vi "Measurement UI.vi"() -> ()   [LabVIEW 2025, in "Automotive Ethernet Bus Monitor UI.lvlib"]
uses:
  Automotive Ethernet Bus Monitor UI.lvlib
  Protocol Layer.ctl
  <vilib>/gRPC/LabVIEW gRPC Library/Shared/grpcId.ctl
  AETH UI Refs.ctl
  <vilib>/Utility/miscctls.llb/LVRowAndColumnUnsignedTypeDef.ctl
  Table Buffer/Get Status.vi
  Table Buffer/Flush Table.vi
  Table Buffer/Create Buffer.vi
  Table Buffer/Destroy Table Buffer.vi
  OOB gRPC Client/OOB gRPC Client.lvlib
  <vilib>/gRPC/LabVIEW gRPC Library/grpc-lvsupport-release.lvlib
panel:
  in  "HELP":bool
  out "IsRestarting?":bool
  out "New Data?":bool
  in  "Clear Packets":bool
  in  "SAVE FORMAT":u16(ring) items=["TDMS", "CSV"]
  in  "INTERFACE NAME":refnum<k21>
  out "TC10 POWER MODE":bool
  in  "TC10":bool
  out "Latest Error":string
  out "STATUS":string
  in  "PAUSE":bool
  out "CAPTURING STREAM":bool
  in  "INTERFACE NAME STRING":string
  in  "ETHERNET MODE IN":i32(ring) items=["Automotive Ethernet", "Standard Ethernet"]
  in  "SAVE TO CSV":bool
  in  "SORT BY":u16(ring) items=["Packet_Number", "Timestamp", "Source", "Destination", "Protocol", "Length", "Data"]
  in  "PATH":path
  in  "FILTER STRING":string
  out "FULL PACKET":string
  out "Packets":string[][](table)=[["10", "11/14/2025 1:57:47 PM", "10.0.0.1", "10.0.0.2", "UDP", "0.821211", "thisisdata"], ["100", "11/14/2025 1:57:47 PM", "10.0.0.1", "10.0.0.2", "UDP", "0.956516", "thisisdata"], ["1002", "11/14/2025 1:57:47 PM", "10.0.0.1", "10.0.0.2", "UDP", "0.960987", "thisisdata"], ["1007", "11/14/2025 1:57:47 PM", "10.0.0.1", "10.0.0.2", "UDP", "0.867598", "thisisdata"], ["1009", "11/14/2025 1:57:47 PM", "10.0.0.1", "10.0.0.2", "UDP", "0.839638", "thisisdata"], ["101", "11/14/2025 1:57:47 PM", "10.0.0.1", "10.0.0.2", "UDP", "0.891709", "thisisdata"], ["1012", "11/14/2025 1:57:47 PM", "10.0.0.1", "10.0.0.2", "UDP", "0.969576", "thisisdata"], ["1017", "11/14/2025 1:57:47 PM", "10.0.0.1", "10.0.0.2", "UDP", "0.871748", "thisisdata"], ["1021", "11/14/2025 1:57:47 PM", "10.0.0.1", "10.0.0.2", "UDP", "0.904588", "thisisdata"], ["1026", "11/14/2025 1:57:47 PM", "10.0.0.1", "10.0.0.2", "UDP", "0.986150", "thisisdata"], ["1027", "11/14/2025 1:57:47 PM", "10.0.0.1", "10.0.0.2", "UDP", "0.775009", "thisisdata"], ["1028", "11/14/2025 1:57:47 PM", "10.0.0.1", "10.0.0.2", "UDP", "0.817026", "thisisdata"], ["1036", "11/14/2025 1:57:47 PM", "10.0.0.1", "10.0.0.2", "UDP", "0.839495", "thisisdata"], ["1038", "11/14/2025 1:57:47 PM", "10.0.0.1", "10.0.0.2", "UDP", "0.847314", "thisisdata"], ["1044", "11/14/2025 1:57:47 PM", "10.0.0.1", "10.0.0.2", "UDP", "0.793260", "thisisdata"], ["1048", "11/14/2025 1:57:47 PM", "10.0.0.1", "10.0.0.2", "UDP", "0.742047", "thisisdata"], ["1049", "11/14/2025 1:57:47 PM", "10.0.0.1", "10.0.0.2", "UDP", "0.771430", "thisisdata"], ["1051", "11/14/2025 1:57:47 PM", "10.0.0.1", "10.0.0.2", "UDP", "0.889463", "thisisdata"], ["1052", "11/14/2025 1:57:47 PM", "10.0.0.1", "10.0.0.2", "UDP", "0.702476", "thisisdata"], ["1053", "11/14/2025 1:57:47 PM", "10.0.0.1", "10.0.0.2", "UDP", "0.943543", "thisisdata"], ["1055", "11/14/2025 1:57:47 PM", "10.0.0.1", "10.0.0.2", "UDP", "0.912358", "thisisdata"], ["1062", "11/14/2025 1:57:47 PM", "10.0.0.1", "10.0.0.2", "UDP", "0.883876", "thisisdata"], ["1065", "11/14/2025 1:57:47 PM", "10.0.0.1", "10.0.0.2", "UDP", "0.998758", "thisisdata"], ["1066", "11/14/2025 1:57:47 PM", "10.0.0.1", "10.0.0.2", "UDP", "0.980816", "thisisdata"], ["1067", "11/14/2025 1:57:47 PM", "10.0.0.1", "10.0.0.2", "UDP", "0.862874", "thisisdata"], ["1074", "11/14/2025 1:57:47 PM", "10.0.0.1", "10.0.0.2", "UDP", "0.985200", "thisisdata"], ["1075", "11/14/2025 1:57:47 PM", "10.0.0.1", "10.0.0.2", "UDP", "0.895925", "thisisdata"], ["108", "11/14/2025 1:57:47 PM", "10.0.0.1", "10.0.0.2", "UDP", "0.746068", "thisisdata"], ["1083", "11/14/2025 1:57:47 PM", "10.0.0.1", "10.0.0.2", "UDP", "0.976636", "thisisdata"], ["1084", "11/14/2025 1:57:47 PM", "10.0.0.1", "10.0.0.2", "UDP", "0.746952", "thisisdata"], ["1086", "11/14/2025 1:57:47 PM", "10.0.0.1", "10.0.0.2", "UDP", "0.772755", "thisisdata"], ["1088", "11/14/2025 1:57:47 PM", "10.0.0.1", "10.0.0.2", "UDP", "0.942784", "thisisdata"], ["1090", "11/14/2025 1:57:47 PM", "10.0.0.1", "10.0.0.2", "UDP", "0.927067", "thisisdata"], ["1092", "11/14/2025 1:57:47 PM", "10.0.0.1", "10.0.0.2", "UDP", "0.875037", "thisisdata"], ["11", "11/14/2025 1:57:47 PM", "10.0.0.1", "10.0.0.2", "UDP", "0.939175", "thisisdata"], ["1101", "11/14/2025 1:57:47 PM", "10.0.0.1", "10.0.0.2", "UDP", "0.730371", "thisisdata"], ["1102", "11/14/2025 1:57:47 PM", "10.0.0.1", "10.0.0.2", "UDP", "0.711041", "thisisdata"], ["1103", "11/14/2025 1:57:47 PM", "10.0.0.1", "10.0.0.2", "UDP", "0.802089", "thisisdata"], ["1104", "11/14/2025 1:57:47 PM", "10.0.0.1", "10.0.0.2", "UDP", "0.975316", "thisisdata"], ["1108", "11/14/2025 1:57:47 PM", "10.0.0.1", "10.0.0.2", "UDP", "0.840307", "thisisdata"], ["1111", "11/14/2025 1:57:47 PM", "10.0.0.1", "10.0.0.2", "UDP", "0.734069", "thisisdata"], ["1113", "11/14/2025 1:57:47 PM", "10.0.0.1", "10.0.0.2", "UDP", "0.897764", "thisisdata"], ["1114", "11/14/2025 1:57:47 PM", "10.0.0.1", "10.0.0.2", "UDP", "0.704577", "thisisdata"], ["1115", "11/14/2025 1:57:47 PM", "10.0.0.1", "10.0.0.2", "UDP", "0.831595", "thisisdata"], ["1123", "11/14/2025 1:57:47 PM", "10.0.0.1", "10.0.0.2", "UDP", "0.869848", "thisisdata"], ["1130", "11/14/2025 1:57:47 PM", "10.0.0.1", "10.0.0.2", "UDP", "0.848458", "thisisdata"], ["1131", "11/14/2025 1:57:47 PM", "10.0.0.1", "10.0.0.2", "UDP", "0.914476", "thisisdata"], ["1139", "11/14/2025 1:57:47 PM", "10.0.0.1", "10.0.0.2", "UDP", "0.851881", "thisisdata"], ["1142", "11/14/2025 1:57:47 PM", "10.0.0.1", "10.0.0.2", "UDP", "0.781918", "thisisdata"], ["1148", "11/14/2025 1:57:47 PM", "10.0.0.1", "10.0.0.2", "UDP", "0.839308", "thisisdata"], ["115", "11/14/2025 1:57:47 PM", "10.0.0.1", "10.0.0.2", "UDP", "0.824463", "thisisdata"], ["1153", "11/14/2025 1:57:47 PM", "10.0.0.1", "10.0.0.2", "UDP", "0.762073", "thisisdata"], ["116", "11/14/2025 1:57:47 PM", "10.0.0.1", "10.0.0.2", "UDP", "0.718284", "thisisdata"], ["1164", "11/14/2025 1:57:47 PM", "10.0.0.1", "10.0.0.2", "UDP", "0.901802", "thisisdata"], ["1165", "11/14/2025 1:57:47 PM", "10.0.0.1", "10.0.0.2", "UDP", "0.782467", "thisisdata"], ["1168", "11/14/2025 1:57:47 PM", "10.0.0.1", "10.0.0.2", "UDP", "0.901873", "thisisdata"], ["1177", "11/14/2025 1:57:47 PM", "10.0.0.1", "10.0.0.2", "UDP", "0.889595", "thisisdata"], ["118", "11/14/2025 1:57:47 PM", "10.0.0.1", "10.0.0.2", "UDP", "0.966309", "thisisdata"], ["1181", "11/14/2025 1:57:47 PM", "10.0.0.1", "10.0.0.2", "UDP", "0.741139", "thisisdata"], ["1182", "11/14/2025 1:57:47 PM", "10.0.0.1", "10.0.0.2", "UDP", "0.954023", "thisisdata"], ["1183", "11/14/2025 1:57:47 PM", "10.0.0.1", "10.0.0.2", "UDP", "0.881562", "thisisdata"], ["1184", "11/14/2025 1:57:47 PM", "10.0.0.1", "10.0.0.2", "UDP", "0.852993", "thisisdata"], ["1185", "11/14/2025 1:57:47 PM", "10.0.0.1", "10.0.0.2", "UDP", "0.885773", "thisisdata"], ["1187", "11/14/2025 1:57:47 PM", "10.0.0.1", "10.0.0.2", "UDP", "0.801737", "thisisdata"], ["1195", "11/14/2025 1:57:47 PM", "10.0.0.1", "10.0.0.2", "UDP", "0.790347", "thisisdata"], ["1196", "11/14/2025 1:57:47 PM", "10.0.0.1", "10.0.0.2", "UDP", "0.864754", "thisisdata"], ["1197", "11/14/2025 1:57:47 PM", "10.0.0.1", "10.0.0.2", "UDP", "0.709221", "thisisdata"], ["121", "11/14/2025 1:57:47 PM", "10.0.0.1", "10.0.0.2", "UDP", "0.913497", "thisisdata"], ["1211", "11/14/2025 1:57:47 PM", "10.0.0.1", "10.0.0.2", "UDP", "0.965122", "thisisdata"], ["1213", "11/14/2025 1:57:47 PM", "10.0.0.1", "10.0.0.2", "UDP", "0.973075", "thisisdata"], ["1218", "11/14/2025 1:57:47 PM", "10.0.0.1", "10.0.0.2", "UDP", "0.904226", "thisisdata"], ["1222", "11/14/2025 1:57:47 PM", "10.0.0.1", "10.0.0.2", "UDP", "0.828121", "thisisdata"], ["1225", "11/14/2025 1:57:47 PM", "10.0.0.1", "10.0.0.2", "UDP", "0.730012", "thisisdata"], ["1226", "11/14/2025 1:57:47 PM", "10.0.0.1", "10.0.0.2", "UDP", "0.762505", "thisisdata"], ["123", "11/14/2025 1:57:47 PM", "10.0.0.1", "10.0.0.2", "UDP", "0.900157", "thisisdata"], ["1230", "11/14/2025 1:57:47 PM", "10.0.0.1", "10.0.0.2", "UDP", "0.958830", "thisisdata"], ["1231", "11/14/2025 1:57:47 PM", "10.0.0.1", "10.0.0.2", "UDP", "0.727490", "thisisdata"], ["1232", "11/14/2025 1:57:47 PM", "10.0.0.1", "10.0.0.2", "UDP", "0.913030", "thisisdata"], ["1234", "11/14/2025 1:57:47 PM", "10.0.0.1", "10.0.0.2", "UDP", "0.711353", "thisisdata"], ["1237", "11/14/2025 1:57:47 PM", "10.0.0.1", "10.0.0.2", "UDP", "0.704839", "thisisdata"], ["1240", "11/14/2025 1:57:47 PM", "10.0.0.1", "10.0.0.2", "UDP", "0.808493", "thisisdata"], ["1241", "11/14/2025 1:57:47 PM", "10.0.0.1", "10.0.0.2", "UDP", "0.750334", "thisisdata"], ["1242", "11/14/2025 1:57:47 PM", "10.0.0.1", "10.0.0.2", "UDP", "0.953795", "thisisdata"], ["1243", "11/14/2025 1:57:47 PM", "10.0.0.1", "10.0.0.2", "UDP", "0.914837", "thisisdata"], ["125", "11/14/2025 1:57:47 PM", "10.0.0.1", "10.0.0.2", "UDP", "0.850827", "thisisdata"], ["1252", "11/14/2025 1:57:47 PM", "10.0.0.1", "10.0.0.2", "UDP", "0.889690", "thisisdata"], ["1253", "11/14/2025 1:57:47 PM", "10.0.0.1", "10.0.0.2", "UDP", "0.800545", "thisisdata"], ["1255", "11/14/2025 1:57:47 PM", "10.0.0.1", "10.0.0.2", "UDP", "0.813802", "thisisdata"], ["1262", "11/14/2025 1:57:47 PM", "10.0.0.1", "10.0.0.2", "UDP", "0.882839", "thisisdata"], ["1265", "11/14/2025 1:57:47 PM", "10.0.0.1", "10.0.0.2", "UDP", "0.898409", "thisisdata"], ["127", "11/14/2025 1:57:47 PM", "10.0.0.1", "10.0.0.2", "UDP", "0.713807", "thisisdata"], ["1275", "11/14/2025 1:57:47 PM", "10.0.0.1", "10.0.0.2", "UDP", "0.972156", "thisisdata"], ["1284", "11/14/2025 1:57:47 PM", "10.0.0.1", "10.0.0.2", "UDP", "0.978269", "thisisdata"], ["1289", "11/14/2025 1:57:47 PM", "10.0.0.1", "10.0.0.2", "UDP", "0.740155", "thisisdata"], ["1299", "11/14/2025 1:57:47 PM", "10.0.0.1", "10.0.0.2", "UDP", "0.953843", "thisisdata"], ["13", "11/14/2025 1:57:47 PM", "10.0.0.1", "10.0.0.2", "UDP", "0.842815", "thisisdata"], ["1301", "11/14/2025 1:57:47 PM", "10.0.0.1", "10.0.0.2", "UDP", "0.879611", "thisisdata"], ["1302", "11/14/2025 1:57:47 PM", "10.0.0.1", "10.0.0.2", "UDP", "0.945983", "thisisdata"], ["1303", "11/14/2025 1:57:47 PM", "10.0.0.1", "10.0.0.2", "UDP", "0.755170", "thisisdata"], ["1307", "11/14/2025 1:57:47 PM", "10.0.0.1", "10.0.0.2", "UDP", "0.773780", "thisisdata"], ["1312", "11/14/2025 1:57:47 PM", "10.0.0.1", "10.0.0.2", "UDP", "0.814087", "thisisdata"], ["1314", "11/14/2025 1:57:47 PM", "10.0.0.1", "10.0.0.2", "UDP", "0.980063", "thisisdata"], ["1317", "11/14/2025 1:57:47 PM", "10.0.0.1", "10.0.0.2", "UDP", "0.829011", "thisisdata"], ["1320", "11/14/2025 1:57:47 PM", "10.0.0.1", "10.0.0.2", "UDP", "0.758120", "thisisdata"], ["1321", "11/14/2025 1:57:47 PM", "10.0.0.1", "10.0.0.2", "UDP", "0.759463", "thisisdata"], ["1322", "11/14/2025 1:57:47 PM", "10.0.0.1", "10.0.0.2", "UDP", "0.824116", "thisisdata"], ["1323", "11/14/2025 1:57:47 PM", "10.0.0.1", "10.0.0.2", "UDP", "0.762172", "thisisdata"], ["1324", "11/14/2025 1:57:47 PM", "10.0.0.1", "10.0.0.2", "UDP", "0.885589", "thisisdata"], ["1330", "11/14/2025 1:57:47 PM", "10.0.0.1", "10.0.0.2", "UDP", "0.942420", "thisisdata"], ["1333", "11/14/2025 1:57:47 PM", "10.0.0.1", "10.0.0.2", "UDP", "0.798878", "thisisdata"], ["1338", "11/14/2025 1:57:47 PM", "10.0.0.1", "10.0.0.2", "UDP", "0.748441", "thisisdata"], ["134", "11/14/2025 1:57:47 PM", "10.0.0.1", "10.0.0.2", "UDP", "0.739118", "thisisdata"], ["1341", "11/14/2025 1:57:47 PM", "10.0.0.1", "10.0.0.2", "UDP", "0.912641", "thisisdata"], ["1342", "11/14/2025 1:57:47 PM", "10.0.0.1", "10.0.0.2", "UDP", "0.833794", "thisisdata"], ["1346", "11/14/2025 1:57:47 PM", "10.0.0.1", "10.0.0.2", "UDP", "0.938173", "thisisdata"], ["1348", "11/14/2025 1:57:47 PM", "10.0.0.1", "10.0.0.2", "UDP", "0.703225", "thisisdata"], ["1349", "11/14/2025 1:57:47 PM", "10.0.0.1", "10.0.0.2", "UDP", "0.962230", "thisisdata"], ["1351", "11/14/2025 1:57:47 PM", "10.0.0.1", "10.0.0.2", "UDP", "0.923262", "thisisdata"], ["1357", "11/14/2025 1:57:47 PM", "10.0.0.1", "10.0.0.2", "UDP", "0.977014", "thisisdata"], ["1358", "11/14/2025 1:57:47 PM", "10.0.0.1", "10.0.0.2", "UDP", "0.904471", "thisisdata"], ["1360", "11/14/2025 1:57:47 PM", "10.0.0.1", "10.0.0.2", "UDP", "0.840541", "thisisdata"], ["1364", "11/14/2025 1:57:47 PM", "10.0.0.1", "10.0.0.2", "UDP", "0.759527", "thisisdata"], ["1367", "11/14/2025 1:57:47 PM", "10.0.0.1", "10.0.0.2", "UDP", "0.926483", "thisisdata"], ["1369", "11/14/2025 1:57:47 PM", "10.0.0.1", "10.0.0.2", "UDP", "0.897696", "thisisdata"], ["1371", "11/14/2025 1:57:47 PM", "10.0.0.1", "10.0.0.2", "UDP", "0.987694", "thisisdata"], ["1374", "11/14/2025 1:57:47 PM", "10.0.0.1", "10.0.0.2", "UDP", "0.795706", "thisisdata"], ["1377", "11/14/2025 1:57:47 PM", "10.0.0.1", "10.0.0.2", "UDP", "0.927883", "thisisdata"], ["1378", "11/14/2025 1:57:47 PM", "10.0.0.1", "10.0.0.2", "UDP", "0.986175", "thisisdata"], ["1379", "11/14/2025 1:57:47 PM", "10.0.0.1", "10.0.0.2", "UDP", "0.716053", "thisisdata"], ["138", "11/14/2025 1:57:47 PM", "10.0.0.1", "10.0.0.2", "UDP", "0.961495", "thisisdata"], ["1381", "11/14/2025 1:57:47 PM", "10.0.0.1", "10.0.0.2", "UDP", "0.839552", "thisisdata"], ["1382", "11/14/2025 1:57:47 PM", "10.0.0.1", "10.0.0.2", "UDP", "0.914187", "thisisdata"], ["1388", "11/14/2025 1:57:47 PM", "10.0.0.1", "10.0.0.2", "UDP", "0.890783", "thisisdata"], ["1390", "11/14/2025 1:57:47 PM", "10.0.0.1", "10.0.0.2", "UDP", "0.913426", "thisisdata"], ["1391", "11/14/2025 1:57:47 PM", "10.0.0.1", "10.0.0.2", "UDP", "0.758421", "thisisdata"], ["1394", "11/14/2025 1:57:47 PM", "10.0.0.1", "10.0.0.2", "UDP", "0.884168", "thisisdata"], ["1395", "11/14/2025 1:57:47 PM", "10.0.0.1", "10.0.0.2", "UDP", "0.773979", "thisisdata"], ["1397", "11/14/2025 1:57:47 PM", "10.0.0.1", "10.0.0.2", "UDP", "0.827235", "thisisdata"], ["14", "11/14/2025 1:57:47 PM", "10.0.0.1", "10.0.0.2", "UDP", "0.839466", "thisisdata"], ["1403", "11/14/2025 1:57:47 PM", "10.0.0.1", "10.0.0.2", "UDP", "0.889704", "thisisdata"], ["1411", "11/14/2025 1:57:47 PM", "10.0.0.1", "10.0.0.2", "UDP", "0.967881", "thisisdata"], ["1417", "11/14/2025 1:57:47 PM", "10.0.0.1", "10.0.0.2", "UDP", "0.962037", "thisisdata"], ["1418", "11/14/2025 1:57:47 PM", "10.0.0.1", "10.0.0.2", "UDP", "0.951923", "thisisdata"], ["1419", "11/14/2025 1:57:47 PM", "10.0.0.1", "10.0.0.2", "UDP", "0.912131", "thisisdata"], ["142", "11/14/2025 1:57:47 PM", "10.0.0.1", "10.0.0.2", "UDP", "0.900485", "thisisdata"], ["1421", "11/14/2025 1:57:47 PM", "10.0.0.1", "10.0.0.2", "UDP", "0.972293", "thisisdata"], ["1428", "11/14/2025 1:57:47 PM", "10.0.0.1", "10.0.0.2", "UDP", "0.706623", "thisisdata"], ["143", "11/14/2025 1:57:47 PM", "10.0.0.1", "10.0.0.2", "UDP", "0.862774", "thisisdata"], ["1430", "11/14/2025 1:57:47 PM", "10.0.0.1", "10.0.0.2", "UDP", "0.831932", "thisisdata"], ["1432", "11/14/2025 1:57:47 PM", "10.0.0.1", "10.0.0.2", "UDP", "0.955880", "thisisdata"], ["1434", "11/14/2025 1:57:47 PM", "10.0.0.1", "10.0.0.2", "UDP", "0.885487", "thisisdata"], ["1436", "11/14/2025 1:57:47 PM", "10.0.0.1", "10.0.0.2", "UDP", "0.804128", "thisisdata"], ["144", "11/14/2025 1:57:47 PM", "10.0.0.1", "10.0.0.2", "UDP", "0.837449", "thisisdata"], ["1440", "11/14/2025 1:57:47 PM", "10.0.0.1", "10.0.0.2", "UDP", "0.973148", "thisisdata"], ["1447", "11/14/2025 1:57:47 PM", "10.0.0.1", "10.0.0.2", "UDP", "0.718230", "thisisdata"], ["1449", "11/14/2025 1:57:47 PM", "10.0.0.1", "10.0.0.2", "UDP", "0.724932", "thisisdata"], ["145", "11/14/2025 1:57:47 PM", "10.0.0.1", "10.0.0.2", "UDP", "0.834936", "thisisdata"], ["1453", "11/14/2025 1:57:47 PM", "10.0.0.1", "10.0.0.2", "UDP", "0.709100", "thisisdata"], ["1457", "11/14/2025 1:57:47 PM", "10.0.0.1", "10.0.0.2", "UDP", "0.785225", "thisisdata"], ["146", "11/14/2025 1:57:47 PM", "10.0.0.1", "10.0.0.2", "UDP", "0.967161", "thisisdata"], ["1467", "11/14/2025 1:57:47 PM", "10.0.0.1", "10.0.0.2", "UDP", "0.721965", "thisisdata"], ["1468", "11/14/2025 1:57:47 PM", "10.0.0.1", "10.0.0.2", "UDP", "0.994270", "thisisdata"], ["1469", "11/14/2025 1:57:47 PM", "10.0.0.1", "10.0.0.2", "UDP", "0.848087", "thisisdata"], ["147", "11/14/2025 1:57:47 PM", "10.0.0.1", "10.0.0.2", "UDP", "0.777765", "thisisdata"], ["1473", "11/14/2025 1:57:47 PM", "10.0.0.1", "10.0.0.2", "UDP", "0.959502", "thisisdata"], ["1474", "11/14/2025 1:57:47 PM", "10.0.0.1", "10.0.0.2", "UDP", "0.934426", "thisisdata"], ["1475", "11/14/2025 1:57:47 PM", "10.0.0.1", "10.0.0.2", "UDP", "0.755909", "thisisdata"], ["1480", "11/14/2025 1:57:47 PM", "10.0.0.1", "10.0.0.2", "UDP", "0.947402", "thisisdata"], ["1482", "11/14/2025 1:57:47 PM", "10.0.0.1", "10.0.0.2", "UDP", "0.966904", "thisisdata"], ["1488", "11/14/2025 1:57:47 PM", "10.0.0.1", "10.0.0.2", "UDP", "0.717426", "thisisdata"], ["1494", "11/14/2025 1:57:47 PM", "10.0.0.1", "10.0.0.2", "UDP", "0.937831", "thisisdata"], ["1496", "11/14/2025 1:57:47 PM", "10.0.0.1", "10.0.0.2", "UDP", "0.872401", "thisisdata"], ["1497", "11/14/2025 1:57:47 PM", "10.0.0.1", "10.0.0.2", "UDP", "0.814240", "thisisdata"], ["1498", "11/14/2025 1:57:47 PM", "10.0.0.1", "10.0.0.2", "UDP", "0.750281", "thisisdata"], ["151", "11/14/2025 1:57:47 PM", "10.0.0.1", "10.0.0.2", "UDP", "0.875864", "thisisdata"], ["152", "11/14/2025 1:57:47 PM", "10.0.0.1", "10.0.0.2", "UDP", "0.771317", "thisisdata"], ["153", "11/14/2025 1:57:47 PM", "10.0.0.1", "10.0.0.2", "UDP", "0.839422", "thisisdata"], ["156", "11/14/2025 1:57:47 PM", "10.0.0.1", "10.0.0.2", "UDP", "0.729712", "thisisdata"], ["158", "11/14/2025 1:57:47 PM", "10.0.0.1", "10.0.0.2", "UDP", "0.878224", "thisisdata"], ["159", "11/14/2025 1:57:47 PM", "10.0.0.1", "10.0.0.2", "UDP", "0.963331", "thisisdata"], ["16", "11/14/2025 1:57:47 PM", "10.0.0.1", "10.0.0.2", "UDP", "0.706402", "thisisdata"], ["160", "11/14/2025 1:57:47 PM", "10.0.0.1", "10.0.0.2", "UDP", "0.803364", "thisisdata"], ["161", "11/14/2025 1:57:47 PM", "10.0.0.1", "10.0.0.2", "UDP", "0.841035", "thisisdata"], ["162", "11/14/2025 1:57:47 PM", "10.0.0.1", "10.0.0.2", "UDP", "0.815937", "thisisdata"], ["171", "11/14/2025 1:57:47 PM", "10.0.0.1", "10.0.0.2", "UDP", "0.923770", "thisisdata"], ["175", "11/14/2025 1:57:47 PM", "10.0.0.1", "10.0.0.2", "UDP", "0.775138", "thisisdata"], ["182", "11/14/2025 1:57:47 PM", "10.0.0.1", "10.0.0.2", "UDP", "0.769656", "thisisdata"], ["183", "11/14/2025 1:57:47 PM", "10.0.0.1", "10.0.0.2", "UDP", "0.886119", "thisisdata"], ["184", "11/14/2025 1:57:47 PM", "10.0.0.1", "10.0.0.2", "UDP", "0.717707", "thisisdata"], ["186", "11/14/2025 1:57:47 PM", "10.0.0.1", "10.0.0.2", "UDP", "0.963742", "thisisdata"], ["189", "11/14/2025 1:57:47 PM", "10.0.0.1", "10.0.0.2", "UDP", "0.822883", "thisisdata"], ["204", "11/14/2025 1:57:47 PM", "10.0.0.1", "10.0.0.2", "UDP", "0.812997", "thisisdata"], ["211", "11/14/2025 1:57:47 PM", "10.0.0.1", "10.0.0.2", "UDP", "0.819247", "thisisdata"], ["215", "11/14/2025 1:57:47 PM", "10.0.0.1", "10.0.0.2", "UDP", "0.723501", "thisisdata"], ["218", "11/14/2025 1:57:47 PM", "10.0.0.1", "10.0.0.2", "UDP", "0.817730", "thisisdata"], ["222", "11/14/2025 1:57:47 PM", "10.0.0.1", "10.0.0.2", "UDP", "0.952346", "thisisdata"], ["225", "11/14/2025 1:57:47 PM", "10.0.0.1", "10.0.0.2", "UDP", "0.939892", "thisisdata"], ["226", "11/14/2025 1:57:47 PM", "10.0.0.1", "10.0.0.2", "UDP", "0.992709", "thisisdata"], ["235", "11/14/2025 1:57:47 PM", "10.0.0.1", "10.0.0.2", "UDP", "0.941276", "thisisdata"], ["246", "11/14/2025 1:57:47 PM", "10.0.0.1", "10.0.0.2", "UDP", "0.904690", "thisisdata"], ["25", "11/14/2025 1:57:47 PM", "10.0.0.1", "10.0.0.2", "UDP", "0.910103", "thisisdata"], ["251", "11/14/2025 1:57:47 PM", "10.0.0.1", "10.0.0.2", "UDP", "0.720603", "thisisdata"], ["252", "11/14/2025 1:57:47 PM", "10.0.0.1", "10.0.0.2", "UDP", "0.978412", "thisisdata"], ["253", "11/14/2025 1:57:47 PM", "10.0.0.1", "10.0.0.2", "UDP", "0.859802", "thisisdata"], ["257", "11/14/2025 1:57:47 PM", "10.0.0.1", "10.0.0.2", "UDP", "0.706716", "thisisdata"], ["265", "11/14/2025 1:57:47 PM", "10.0.0.1", "10.0.0.2", "UDP", "0.954216", "thisisdata"], ["266", "11/14/2025 1:57:47 PM", "10.0.0.1", "10.0.0.2", "UDP", "0.978586", "thisisdata"], ["268", "11/14/2025 1:57:47 PM", "10.0.0.1", "10.0.0.2", "UDP", "0.728359", "thisisdata"], ["269", "11/14/2025 1:57:47 PM", "10.0.0.1", "10.0.0.2", "UDP", "0.805801", "thisisdata"], ["27", "11/14/2025 1:57:47 PM", "10.0.0.1", "10.0.0.2", "UDP", "0.890670", "thisisdata"], ["270", "11/14/2025 1:57:47 PM", "10.0.0.1", "10.0.0.2", "UDP", "0.730876", "thisisdata"], ["271", "11/14/2025 1:57:47 PM", "10.0.0.1", "10.0.0.2", "UDP", "0.964321", "thisisdata"], ["273", "11/14/2025 1:57:47 PM", "10.0.0.1", "10.0.0.2", "UDP", "0.822445", "thisisdata"], ["280", "11/14/2025 1:57:47 PM", "10.0.0.1", "10.0.0.2", "UDP", "0.805915", "thisisdata"], ["282", "11/14/2025 1:57:47 PM", "10.0.0.1", "10.0.0.2", "UDP", "0.995119", "thisisdata"], ["285", "11/14/2025 1:57:47 PM", "10.0.0.1", "10.0.0.2", "UDP", "0.702493", "thisisdata"], ["287", "11/14/2025 1:57:47 PM", "10.0.0.1", "10.0.0.2", "UDP", "0.895930", "thisisdata"], ["293", "11/14/2025 1:57:47 PM", "10.0.0.1", "10.0.0.2", "UDP", "0.782899", "thisisdata"], ["30", "11/14/2025 1:57:47 PM", "10.0.0.1", "10.0.0.2", "UDP", "0.919602", "thisisdata"], ["302", "11/14/2025 1:57:47 PM", "10.0.0.1", "10.0.0.2", "UDP", "0.702472", "thisisdata"], ["303", "11/14/2025 1:57:47 PM", "10.0.0.1", "10.0.0.2", "UDP", "0.776732", "thisisdata"], ["304", "11/14/2025 1:57:47 PM", "10.0.0.1", "10.0.0.2", "UDP", "0.805126", "thisisdata"], ["305", "11/14/2025 1:57:47 PM", "10.0.0.1", "10.0.0.2", "UDP", "0.974208", "thisisdata"], ["306", "11/14/2025 1:57:47 PM", "10.0.0.1", "10.0.0.2", "UDP", "0.799271", "thisisdata"], ["307", "11/14/2025 1:57:47 PM", "10.0.0.1", "10.0.0.2", "UDP", "0.985518", "thisisdata"], ["310", "11/14/2025 1:57:47 PM", "10.0.0.1", "10.0.0.2", "UDP", "0.995978", "thisisdata"], ["311", "11/14/2025 1:57:47 PM", "10.0.0.1", "10.0.0.2", "UDP", "0.987227", "thisisdata"], ["312", "11/14/2025 1:57:47 PM", "10.0.0.1", "10.0.0.2", "UDP", "0.797511", "thisisdata"], ["314", "11/14/2025 1:57:47 PM", "10.0.0.1", "10.0.0.2", "UDP", "0.838158", "thisisdata"], ["316", "11/14/2025 1:57:47 PM", "10.0.0.1", "10.0.0.2", "UDP", "0.898183", "thisisdata"], ["319", "11/14/2025 1:57:47 PM", "10.0.0.1", "10.0.0.2", "UDP", "0.813462", "thisisdata"], ["320", "11/14/2025 1:57:47 PM", "10.0.0.1", "10.0.0.2", "UDP", "0.725049", "thisisdata"], ["322", "11/14/2025 1:57:47 PM", "10.0.0.1", "10.0.0.2", "UDP", "0.954221", "thisisdata"], ["324", "11/14/2025 1:57:47 PM", "10.0.0.1", "10.0.0.2", "UDP", "0.773913", "thisisdata"], ["330", "11/14/2025 1:57:47 PM", "10.0.0.1", "10.0.0.2", "UDP", "0.846395", "thisisdata"], ["331", "11/14/2025 1:57:47 PM", "10.0.0.1", "10.0.0.2", "UDP", "0.868667", "thisisdata"], ["333", "11/14/2025 1:57:47 PM", "10.0.0.1", "10.0.0.2", "UDP", "0.915934", "thisisdata"], ["335", "11/14/2025 1:57:47 PM", "10.0.0.1", "10.0.0.2", "UDP", "0.744820", "thisisdata"], ["344", "11/14/2025 1:57:47 PM", "10.0.0.1", "10.0.0.2", "UDP", "0.737303", "thisisdata"], ["345", "11/14/2025 1:57:47 PM", "10.0.0.1", "10.0.0.2", "UDP", "0.744197", "thisisdata"], ["347", "11/14/2025 1:57:47 PM", "10.0.0.1", "10.0.0.2", "UDP", "0.816133", "thisisdata"], ["35", "11/14/2025 1:57:47 PM", "10.0.0.1", "10.0.0.2", "UDP", "0.980754", "thisisdata"], ["359", "11/14/2025 1:57:47 PM", "10.0.0.1", "10.0.0.2", "UDP", "0.710696", "thisisdata"], ["36", "11/14/2025 1:57:47 PM", "10.0.0.1", "10.0.0.2", "UDP", "0.821418", "thisisdata"], ["361", "11/14/2025 1:57:47 PM", "10.0.0.1", "10.0.0.2", "UDP", "0.810013", "thisisdata"], ["369", "11/14/2025 1:57:47 PM", "10.0.0.1", "10.0.0.2", "UDP", "0.918693", "thisisdata"], ["373", "11/14/2025 1:57:47 PM", "10.0.0.1", "10.0.0.2", "UDP", "0.860255", "thisisdata"], ["376", "11/14/2025 1:57:47 PM", "10.0.0.1", "10.0.0.2", "UDP", "0.749631", "thisisdata"], ["38", "11/14/2025 1:57:47 PM", "10.0.0.1", "10.0.0.2", "UDP", "0.844976", "thisisdata"], ["383", "11/14/2025 1:57:47 PM", "10.0.0.1", "10.0.0.2", "UDP", "0.800813", "thisisdata"], ["384", "11/14/2025 1:57:47 PM", "10.0.0.1", "10.0.0.2", "UDP", "0.765681", "thisisdata"], ["391", "11/14/2025 1:57:47 PM", "10.0.0.1", "10.0.0.2", "UDP", "0.710353", "thisisdata"], ["392", "11/14/2025 1:57:47 PM", "10.0.0.1", "10.0.0.2", "UDP", "0.798826", "thisisdata"], ["393", "11/14/2025 1:57:47 PM", "10.0.0.1", "10.0.0.2", "UDP", "0.888259", "thisisdata"], ["394", "11/14/2025 1:57:47 PM", "10.0.0.1", "10.0.0.2", "UDP", "0.728993", "thisisdata"], ["406", "11/14/2025 1:57:47 PM", "10.0.0.1", "10.0.0.2", "UDP", "0.924575", "thisisdata"], ["408", "11/14/2025 1:57:47 PM", "10.0.0.1", "10.0.0.2", "UDP", "0.827347", "thisisdata"], ["41", "11/14/2025 1:57:47 PM", "10.0.0.1", "10.0.0.2", "UDP", "0.897112", "thisisdata"], ["412", "11/14/2025 1:57:47 PM", "10.0.0.1", "10.0.0.2", "UDP", "0.823947", "thisisdata"], ["414", "11/14/2025 1:57:47 PM", "10.0.0.1", "10.0.0.2", "UDP", "0.706129", "thisisdata"], ["415", "11/14/2025 1:57:47 PM", "10.0.0.1", "10.0.0.2", "UDP", "0.712052", "thisisdata"], ["42", "11/14/2025 1:57:47 PM", "10.0.0.1", "10.0.0.2", "UDP", "0.984320", "thisisdata"], ["421", "11/14/2025 1:57:47 PM", "10.0.0.1", "10.0.0.2", "UDP", "0.790512", "thisisdata"], ["428", "11/14/2025 1:57:47 PM", "10.0.0.1", "10.0.0.2", "UDP", "0.825226", "thisisdata"], ["431", "11/14/2025 1:57:47 PM", "10.0.0.1", "10.0.0.2", "UDP", "0.866616", "thisisdata"], ["433", "11/14/2025 1:57:47 PM", "10.0.0.1", "10.0.0.2", "UDP", "0.906895", "thisisdata"], ["442", "11/14/2025 1:57:47 PM", "10.0.0.1", "10.0.0.2", "UDP", "0.885974", "thisisdata"], ["448", "11/14/2025 1:57:47 PM", "10.0.0.1", "10.0.0.2", "UDP", "0.888818", "thisisdata"], ["453", "11/14/2025 1:57:47 PM", "10.0.0.1", "10.0.0.2", "UDP", "0.742889", "thisisdata"], ["456", "11/14/2025 1:57:47 PM", "10.0.0.1", "10.0.0.2", "UDP", "0.808371", "thisisdata"], ["459", "11/14/2025 1:57:47 PM", "10.0.0.1", "10.0.0.2", "UDP", "0.878908", "thisisdata"], ["461", "11/14/2025 1:57:47 PM", "10.0.0.1", "10.0.0.2", "UDP", "0.935594", "thisisdata"], ["463", "11/14/2025 1:57:47 PM", "10.0.0.1", "10.0.0.2", "UDP", "0.917788", "thisisdata"], ["465", "11/14/2025 1:57:47 PM", "10.0.0.1", "10.0.0.2", "UDP", "0.924728", "thisisdata"], ["467", "11/14/2025 1:57:47 PM", "10.0.0.1", "10.0.0.2", "UDP", "0.802965", "thisisdata"], ["471", "11/14/2025 1:57:47 PM", "10.0.0.1", "10.0.0.2", "UDP", "0.920198", "thisisdata"], ["473", "11/14/2025 1:57:47 PM", "10.0.0.1", "10.0.0.2", "UDP", "0.712752", "thisisdata"], ["48", "11/14/2025 1:57:47 PM", "10.0.0.1", "10.0.0.2", "UDP", "0.894854", "thisisdata"], ["484", "11/14/2025 1:57:47 PM", "10.0.0.1", "10.0.0.2", "UDP", "0.934918", "thisisdata"], ["487", "11/14/2025 1:57:47 PM", "10.0.0.1", "10.0.0.2", "UDP", "0.753021", "thisisdata"], ["489", "11/14/2025 1:57:47 PM", "10.0.0.1", "10.0.0.2", "UDP", "0.794461", "thisisdata"], ["493", "11/14/2025 1:57:47 PM", "10.0.0.1", "10.0.0.2", "UDP", "0.879307", "thisisdata"], ["494", "11/14/2025 1:57:47 PM", "10.0.0.1", "10.0.0.2", "UDP", "0.821176", "thisisdata"], ["496", "11/14/2025 1:57:47 PM", "10.0.0.1", "10.0.0.2", "UDP", "0.808411", "thisisdata"], ["498", "11/14/2025 1:57:47 PM", "10.0.0.1", "10.0.0.2", "UDP", "0.911798", "thisisdata"], ["5", "11/14/2025 1:57:47 PM", "10.0.0.1", "10.0.0.2", "UDP", "0.924127", "thisisdata"], ["501", "11/14/2025 1:57:47 PM", "10.0.0.1", "10.0.0.2", "UDP", "0.946039", "thisisdata"], ["505", "11/14/2025 1:57:47 PM", "10.0.0.1", "10.0.0.2", "UDP", "0.800570", "thisisdata"], ["509", "11/14/2025 1:57:47 PM", "10.0.0.1", "10.0.0.2", "UDP", "0.879202", "thisisdata"], ["511", "11/14/2025 1:57:47 PM", "10.0.0.1", "10.0.0.2", "UDP", "0.707965", "thisisdata"], ["517", "11/14/2025 1:57:47 PM", "10.0.0.1", "10.0.0.2", "UDP", "0.759952", "thisisdata"], ["518", "11/14/2025 1:57:47 PM", "10.0.0.1", "10.0.0.2", "UDP", "0.720618", "thisisdata"], ["520", "11/14/2025 1:57:47 PM", "10.0.0.1", "10.0.0.2", "UDP", "0.806107", "thisisdata"], ["530", "11/14/2025 1:57:47 PM", "10.0.0.1", "10.0.0.2", "UDP", "0.995294", "thisisdata"], ["531", "11/14/2025 1:57:47 PM", "10.0.0.1", "10.0.0.2", "UDP", "0.734341", "thisisdata"], ["538", "11/14/2025 1:57:47 PM", "10.0.0.1", "10.0.0.2", "UDP", "0.791430", "thisisdata"], ["552", "11/14/2025 1:57:47 PM", "10.0.0.1", "10.0.0.2", "UDP", "0.803719", "thisisdata"], ["553", "11/14/2025 1:57:47 PM", "10.0.0.1", "10.0.0.2", "UDP", "0.798672", "thisisdata"], ["555", "11/14/2025 1:57:47 PM", "10.0.0.1", "10.0.0.2", "UDP", "0.718180", "thisisdata"], ["556", "11/14/2025 1:57:47 PM", "10.0.0.1", "10.0.0.2", "UDP", "0.712425", "thisisdata"], ["557", "11/14/2025 1:57:47 PM", "10.0.0.1", "10.0.0.2", "UDP", "0.839688", "thisisdata"], ["561", "11/14/2025 1:57:47 PM", "10.0.0.1", "10.0.0.2", "UDP", "0.973886", "thisisdata"], ["575", "11/14/2025 1:57:47 PM", "10.0.0.1", "10.0.0.2", "UDP", "0.829130", "thisisdata"], ["576", "11/14/2025 1:57:47 PM", "10.0.0.1", "10.0.0.2", "UDP", "0.725344", "thisisdata"], ["579", "11/14/2025 1:57:47 PM", "10.0.0.1", "10.0.0.2", "UDP", "0.857040", "thisisdata"], ["580", "11/14/2025 1:57:47 PM", "10.0.0.1", "10.0.0.2", "UDP", "0.919608", "thisisdata"], ["584", "11/14/2025 1:57:47 PM", "10.0.0.1", "10.0.0.2", "UDP", "0.875136", "thisisdata"], ["585", "11/14/2025 1:57:47 PM", "10.0.0.1", "10.0.0.2", "UDP", "0.791057", "thisisdata"], ["59", "11/14/2025 1:57:47 PM", "10.0.0.1", "10.0.0.2", "UDP", "0.836493", "thisisdata"], ["591", "11/14/2025 1:57:47 PM", "10.0.0.1", "10.0.0.2", "UDP", "0.861319", "thisisdata"], ["592", "11/14/2025 1:57:47 PM", "10.0.0.1", "10.0.0.2", "UDP", "0.916902", "thisisdata"], ["599", "11/14/2025 1:57:47 PM", "10.0.0.1", "10.0.0.2", "UDP", "0.903742", "thisisdata"], ["60", "11/14/2025 1:57:47 PM", "10.0.0.1", "10.0.0.2", "UDP", "0.871553", "thisisdata"], ["603", "11/14/2025 1:57:47 PM", "10.0.0.1", "10.0.0.2", "UDP", "0.905091", "thisisdata"], ["606", "11/14/2025 1:57:47 PM", "10.0.0.1", "10.0.0.2", "UDP", "0.886018", "thisisdata"], ["609", "11/14/2025 1:57:47 PM", "10.0.0.1", "10.0.0.2", "UDP", "0.710266", "thisisdata"], ["610", "11/14/2025 1:57:47 PM", "10.0.0.1", "10.0.0.2", "UDP", "0.785021", "thisisdata"], ["614", "11/14/2025 1:57:47 PM", "10.0.0.1", "10.0.0.2", "UDP", "0.714634", "thisisdata"], ["622", "11/14/2025 1:57:47 PM", "10.0.0.1", "10.0.0.2", "UDP", "0.912282", "thisisdata"], ["624", "11/14/2025 1:57:47 PM", "10.0.0.1", "10.0.0.2", "UDP", "0.890598", "thisisdata"], ["631", "11/14/2025 1:57:47 PM", "10.0.0.1", "10.0.0.2", "UDP", "0.748006", "thisisdata"], ["634", "11/14/2025 1:57:47 PM", "10.0.0.1", "10.0.0.2", "UDP", "0.791920", "thisisdata"], ["64", "11/14/2025 1:57:47 PM", "10.0.0.1", "10.0.0.2", "UDP", "0.967066", "thisisdata"], ["642", "11/14/2025 1:57:47 PM", "10.0.0.1", "10.0.0.2", "UDP", "0.783278", "thisisdata"], ["644", "11/14/2025 1:57:47 PM", "10.0.0.1", "10.0.0.2", "UDP", "0.893851", "thisisdata"], ["65", "11/14/2025 1:57:47 PM", "10.0.0.1", "10.0.0.2", "UDP", "0.809766", "thisisdata"], ["657", "11/14/2025 1:57:47 PM", "10.0.0.1", "10.0.0.2", "UDP", "0.710376", "thisisdata"], ["660", "11/14/2025 1:57:47 PM", "10.0.0.1", "10.0.0.2", "UDP", "0.897561", "thisisdata"], ["661", "11/14/2025 1:57:47 PM", "10.0.0.1", "10.0.0.2", "UDP", "0.907407", "thisisdata"], ["668", "11/14/2025 1:57:47 PM", "10.0.0.1", "10.0.0.2", "UDP", "0.970645", "thisisdata"], ["669", "11/14/2025 1:57:47 PM", "10.0.0.1", "10.0.0.2", "UDP", "0.994801", "thisisdata"], ["671", "11/14/2025 1:57:47 PM", "10.0.0.1", "10.0.0.2", "UDP", "0.957190", "thisisdata"], ["672", "11/14/2025 1:57:47 PM", "10.0.0.1", "10.0.0.2", "UDP", "0.834875", "thisisdata"], ["683", "11/14/2025 1:57:47 PM", "10.0.0.1", "10.0.0.2", "UDP", "0.893810", "thisisdata"], ["692", "11/14/2025 1:57:47 PM", "10.0.0.1", "10.0.0.2", "UDP", "0.716870", "thisisdata"], ["698", "11/14/2025 1:57:47 PM", "10.0.0.1", "10.0.0.2", "UDP", "0.812164", "thisisdata"], ["699", "11/14/2025 1:57:47 PM", "10.0.0.1", "10.0.0.2", "UDP", "0.959842", "thisisdata"], ["700", "11/14/2025 1:57:47 PM", "10.0.0.1", "10.0.0.2", "UDP", "0.726590", "thisisdata"], ["711", "11/14/2025 1:57:47 PM", "10.0.0.1", "10.0.0.2", "UDP", "0.823803", "thisisdata"], ["714", "11/14/2025 1:57:47 PM", "10.0.0.1", "10.0.0.2", "UDP", "0.773208", "thisisdata"], ["718", "11/14/2025 1:57:47 PM", "10.0.0.1", "10.0.0.2", "UDP", "0.768409", "thisisdata"], ["721", "11/14/2025 1:57:47 PM", "10.0.0.1", "10.0.0.2", "UDP", "0.793787", "thisisdata"], ["725", "11/14/2025 1:57:47 PM", "10.0.0.1", "10.0.0.2", "UDP", "0.976198", "thisisdata"], ["730", "11/14/2025 1:57:47 PM", "10.0.0.1", "10.0.0.2", "UDP", "0.885853", "thisisdata"], ["731", "11/14/2025 1:57:47 PM", "10.0.0.1", "10.0.0.2", "UDP", "0.842282", "thisisdata"], ["734", "11/14/2025 1:57:47 PM", "10.0.0.1", "10.0.0.2", "UDP", "0.751845", "thisisdata"], ["735", "11/14/2025 1:57:47 PM", "10.0.0.1", "10.0.0.2", "UDP", "0.775000", "thisisdata"], ["739", "11/14/2025 1:57:47 PM", "10.0.0.1", "10.0.0.2", "UDP", "0.933339", "thisisdata"], ["74", "11/14/2025 1:57:47 PM", "10.0.0.1", "10.0.0.2", "UDP", "0.927019", "thisisdata"], ["740", "11/14/2025 1:57:47 PM", "10.0.0.1", "10.0.0.2", "UDP", "0.862581", "thisisdata"], ["75", "11/14/2025 1:57:47 PM", "10.0.0.1", "10.0.0.2", "UDP", "0.712333", "thisisdata"], ["752", "11/14/2025 1:57:47 PM", "10.0.0.1", "10.0.0.2", "UDP", "0.853785", "thisisdata"], ["754", "11/14/2025 1:57:47 PM", "10.0.0.1", "10.0.0.2", "UDP", "0.961801", "thisisdata"], ["756", "11/14/2025 1:57:47 PM", "10.0.0.1", "10.0.0.2", "UDP", "0.885805", "thisisdata"], ["761", "11/14/2025 1:57:47 PM", "10.0.0.1", "10.0.0.2", "UDP", "0.892997", "thisisdata"], ["762", "11/14/2025 1:57:47 PM", "10.0.0.1", "10.0.0.2", "UDP", "0.981252", "thisisdata"], ["763", "11/14/2025 1:57:47 PM", "10.0.0.1", "10.0.0.2", "UDP", "0.739524", "thisisdata"], ["779", "11/14/2025 1:57:47 PM", "10.0.0.1", "10.0.0.2", "UDP", "0.846841", "thisisdata"], ["782", "11/14/2025 1:57:47 PM", "10.0.0.1", "10.0.0.2", "UDP", "0.960776", "thisisdata"], ["784", "11/14/2025 1:57:47 PM", "10.0.0.1", "10.0.0.2", "UDP", "0.834294", "thisisdata"], ["786", "11/14/2025 1:57:47 PM", "10.0.0.1", "10.0.0.2", "UDP", "0.976165", "thisisdata"], ["794", "11/14/2025 1:57:47 PM", "10.0.0.1", "10.0.0.2", "UDP", "0.738251", "thisisdata"], ["796", "11/14/2025 1:57:47 PM", "10.0.0.1", "10.0.0.2", "UDP", "0.765415", "thisisdata"], ["80", "11/14/2025 1:57:47 PM", "10.0.0.1", "10.0.0.2", "UDP", "0.838034", "thisisdata"], ["804", "11/14/2025 1:57:47 PM", "10.0.0.1", "10.0.0.2", "UDP", "0.832158", "thisisdata"], ["806", "11/14/2025 1:57:47 PM", "10.0.0.1", "10.0.0.2", "UDP", "0.872118", "thisisdata"], ["809", "11/14/2025 1:57:47 PM", "10.0.0.1", "10.0.0.2", "UDP", "0.906668", "thisisdata"], ["811", "11/14/2025 1:57:47 PM", "10.0.0.1", "10.0.0.2", "UDP", "0.765262", "thisisdata"], ["816", "11/14/2025 1:57:47 PM", "10.0.0.1", "10.0.0.2", "UDP", "0.937976", "thisisdata"], ["832", "11/14/2025 1:57:47 PM", "10.0.0.1", "10.0.0.2", "UDP", "0.910402", "thisisdata"], ["844", "11/14/2025 1:57:47 PM", "10.0.0.1", "10.0.0.2", "UDP", "0.916379", "thisisdata"], ["847", "11/14/2025 1:57:47 PM", "10.0.0.1", "10.0.0.2", "UDP", "0.823197", "thisisdata"], ["849", "11/14/2025 1:57:47 PM", "10.0.0.1", "10.0.0.2", "UDP", "0.788440", "thisisdata"], ["851", "11/14/2025 1:57:47 PM", "10.0.0.1", "10.0.0.2", "UDP", "0.842912", "thisisdata"], ["858", "11/14/2025 1:57:47 PM", "10.0.0.1", "10.0.0.2", "UDP", "0.800903", "thisisdata"], ["859", "11/14/2025 1:57:47 PM", "10.0.0.1", "10.0.0.2", "UDP", "0.976923", "thisisdata"], ["86", "11/14/2025 1:57:47 PM", "10.0.0.1", "10.0.0.2", "UDP", "0.854198", "thisisdata"], ["861", "11/14/2025 1:57:47 PM", "10.0.0.1", "10.0.0.2", "UDP", "0.815290", "thisisdata"], ["862", "11/14/2025 1:57:47 PM", "10.0.0.1", "10.0.0.2", "UDP", "0.953745", "thisisdata"], ["863", "11/14/2025 1:57:47 PM", "10.0.0.1", "10.0.0.2", "UDP", "0.960371", "thisisdata"], ["864", "11/14/2025 1:57:47 PM", "10.0.0.1", "10.0.0.2", "UDP", "0.852174", "thisisdata"], ["865", "11/14/2025 1:57:47 PM", "10.0.0.1", "10.0.0.2", "UDP", "0.969242", "thisisdata"], ["870", "11/14/2025 1:57:47 PM", "10.0.0.1", "10.0.0.2", "UDP", "0.947803", "thisisdata"], ["871", "11/14/2025 1:57:47 PM", "10.0.0.1", "10.0.0.2", "UDP", "0.985852", "thisisdata"], ["874", "11/14/2025 1:57:47 PM", "10.0.0.1", "10.0.0.2", "UDP", "0.745448", "thisisdata"], ["879", "11/14/2025 1:57:47 PM", "10.0.0.1", "10.0.0.2", "UDP", "0.828622", "thisisdata"], ["881", "11/14/2025 1:57:47 PM", "10.0.0.1", "10.0.0.2", "UDP", "0.709092", "thisisdata"], ["882", "11/14/2025 1:57:47 PM", "10.0.0.1", "10.0.0.2", "UDP", "0.754218", "thisisdata"], ["884", "11/14/2025 1:57:47 PM", "10.0.0.1", "10.0.0.2", "UDP", "0.815853", "thisisdata"], ["887", "11/14/2025 1:57:47 PM", "10.0.0.1", "10.0.0.2", "UDP", "0.873913", "thisisdata"], ["888", "11/14/2025 1:57:47 PM", "10.0.0.1", "10.0.0.2", "UDP", "0.999693", "thisisdata"], ["889", "11/14/2025 1:57:47 PM", "10.0.0.1", "10.0.0.2", "UDP", "0.949421", "thisisdata"], ["89", "11/14/2025 1:57:47 PM", "10.0.0.1", "10.0.0.2", "UDP", "0.867253", "thisisdata"], ["897", "11/14/2025 1:57:47 PM", "10.0.0.1", "10.0.0.2", "UDP", "0.872446", "thisisdata"], ["898", "11/14/2025 1:57:47 PM", "10.0.0.1", "10.0.0.2", "UDP", "0.932192", "thisisdata"], ["899", "11/14/2025 1:57:47 PM", "10.0.0.1", "10.0.0.2", "UDP", "0.896984", "thisisdata"], ["9", "11/14/2025 1:57:47 PM", "10.0.0.1", "10.0.0.2", "UDP", "0.840249", "thisisdata"], ["909", "11/14/2025 1:57:47 PM", "10.0.0.1", "10.0.0.2", "UDP", "0.863075", "thisisdata"], ["91", "11/14/2025 1:57:47 PM", "10.0.0.1", "10.0.0.2", "UDP", "0.974346", "thisisdata"], ["913", "11/14/2025 1:57:47 PM", "10.0.0.1", "10.0.0.2", "UDP", "0.930396", "thisisdata"], ["914", "11/14/2025 1:57:47 PM", "10.0.0.1", "10.0.0.2", "UDP", "0.937608", "thisisdata"], ["918", "11/14/2025 1:57:47 PM", "10.0.0.1", "10.0.0.2", "UDP", "0.813773", "thisisdata"], ["922", "11/14/2025 1:57:47 PM", "10.0.0.1", "10.0.0.2", "UDP", "0.903496", "thisisdata"], ["925", "11/14/2025 1:57:47 PM", "10.0.0.1", "10.0.0.2", "UDP", "0.836203", "thisisdata"], ["93", "11/14/2025 1:57:47 PM", "10.0.0.1", "10.0.0.2", "UDP", "0.992103", "thisisdata"], ["931", "11/14/2025 1:57:47 PM", "10.0.0.1", "10.0.0.2", "UDP", "0.742922", "thisisdata"], ["935", "11/14/2025 1:57:47 PM", "10.0.0.1", "10.0.0.2", "UDP", "0.942935", "thisisdata"], ["936", "11/14/2025 1:57:47 PM", "10.0.0.1", "10.0.0.2", "UDP", "0.731021", "thisisdata"], ["94", "11/14/2025 1:57:47 PM", "10.0.0.1", "10.0.0.2", "UDP", "0.833321", "thisisdata"], ["944", "11/14/2025 1:57:47 PM", "10.0.0.1", "10.0.0.2", "UDP", "0.700170", "thisisdata"], ["945", "11/14/2025 1:57:47 PM", "10.0.0.1", "10.0.0.2", "UDP", "0.795369", "thisisdata"], ["946", "11/14/2025 1:57:47 PM", "10.0.0.1", "10.0.0.2", "UDP", "0.705826", "thisisdata"], ["950", "11/14/2025 1:57:47 PM", "10.0.0.1", "10.0.0.2", "UDP", "0.903245", "thisisdata"], ["956", "11/14/2025 1:57:47 PM", "10.0.0.1", "10.0.0.2", "UDP", "0.772137", "thisisdata"], ["962", "11/14/2025 1:57:47 PM", "10.0.0.1", "10.0.0.2", "UDP", "0.785660", "thisisdata"], ["971", "11/14/2025 1:57:47 PM", "10.0.0.1", "10.0.0.2", "UDP", "0.958167", "thisisdata"], ["973", "11/14/2025 1:57:47 PM", "10.0.0.1", "10.0.0.2", "UDP", "0.941597", "thisisdata"], ["974", "11/14/2025 1:57:47 PM", "10.0.0.1", "10.0.0.2", "UDP", "0.956441", "thisisdata"], ["976", "11/14/2025 1:57:47 PM", "10.0.0.1", "10.0.0.2", "UDP", "0.908337", "thisisdata"], ["977", "11/14/2025 1:57:47 PM", "10.0.0.1", "10.0.0.2", "UDP", "0.752689", "thisisdata"], ["983", "11/14/2025 1:57:47 PM", "10.0.0.1", "10.0.0.2", "UDP", "0.933649", "thisisdata"], ["985", "11/14/2025 1:57:47 PM", "10.0.0.1", "10.0.0.2", "UDP", "0.788836", "thisisdata"], ["987", "11/14/2025 1:57:47 PM", "10.0.0.1", "10.0.0.2", "UDP", "0.979633", "thisisdata"], ["988", "11/14/2025 1:57:47 PM", "10.0.0.1", "10.0.0.2", "UDP", "0.723583", "thisisdata"], ["989", "11/14/2025 1:57:47 PM", "10.0.0.1", "10.0.0.2", "UDP", "0.910875", "thisisdata"], ["99", "11/14/2025 1:57:47 PM", "10.0.0.1", "10.0.0.2", "UDP", "0.869477", "thisisdata"], ["995", "11/14/2025 1:57:47 PM", "10.0.0.1", "10.0.0.2", "UDP", "0.827503", "thisisdata"], ["996", "11/14/2025 1:57:47 PM", "10.0.0.1", "10.0.0.2", "UDP", "0.904767", "thisisdata"], ["999", "11/14/2025 1:57:47 PM", "10.0.0.1", "10.0.0.2", "UDP", "0.952043", "thisisdata"]]
  out "OOB gRPC Port":i32
  out "Protocol Layer":T1
  out "RECEIVED PACKETS":i32
  out "Status Message":string
  out "PAYLOAD":string
  out "Dataframe":string[][](array[string])
  # "CONFIGURATION"
  # "CONTROL"
  # "DATA LAYER"
  # "STATUS"
  # "PACKETS"
  # "PROTOCOL LAYER"
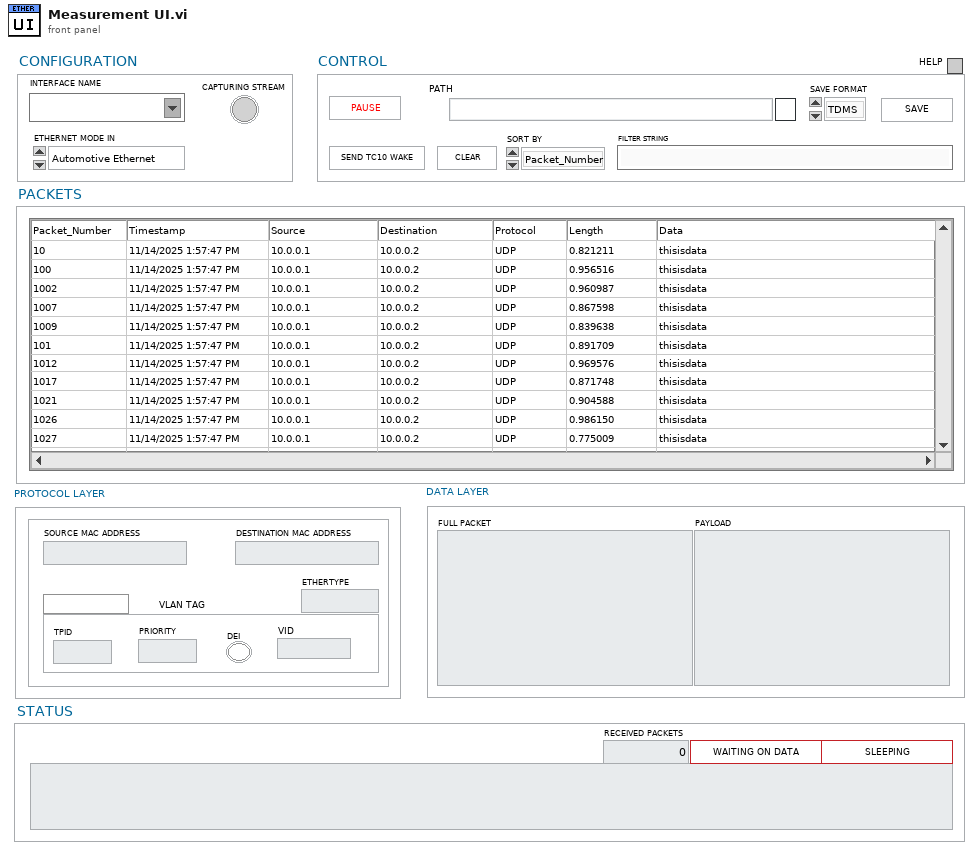
[diagram p1: front panel]
types:
  T1 = typedef "Automotive Ethernet Bus Monitor UI.lvlib/Protocol Layer.ctl" = cluster{"Has VLAN":bool, "VLAN TAG":cluster{"TPID":u16, "PRIORITY":u8, "DEI":bool, "VID":u16}, "SOURCE MAC ADDRESS":string, "DESTINATION MAC ADDRESS":string, "ETHERTYPE":u16}
  T2 = typedef "Automotive Ethernet Bus Monitor UI.lvlib/AETH UI Refs.ctl" = cluster{"Packets":refnum<vi>, "PAUSE":refnum<vi>, "PATH ":refnum<vi>, "SAVE FORMAT":refnum<vi>, "SAVE TO CSV":refnum<vi>, "ETHERNET MODE IN":refnum<vi>, "FILTER STRING":refnum<vi>, "SORT BY":refnum<vi>, "Status Message":refnum<vi>, "INTERFACE NAME":refnum<vi>, "TC10 POWER MODE":refnum<vi>}
  T3 = typedef "grpc-lvsupport-release.lvlib/grpcId.ctl" = u64
  T4 = typedef "LVRowAndColumnUnsignedTypeDef.ctl" = cluster{"Row":u32, "Column":u32}
  T5 = typedef "LVPoint32TypeDef.ctl" = cluster{"Horizontal":i32, "Vertical":i32}
  T6 = typedef "Automotive Ethernet Bus Monitor UI.lvlib/Ethernet Header Cluster.ctl" = cluster{"destination MAC address":cluster{u8, u8, u8, u8, u8, u8}, "source MAC address":cluster{u8, u8, u8, u8, u8, u8}, "Has VLAN Tag":bool, "VLAN Tag":cluster{"TPID":u16, "priority":u8, "DEI":bool, "VID":u16}, "Ethertype":u16}
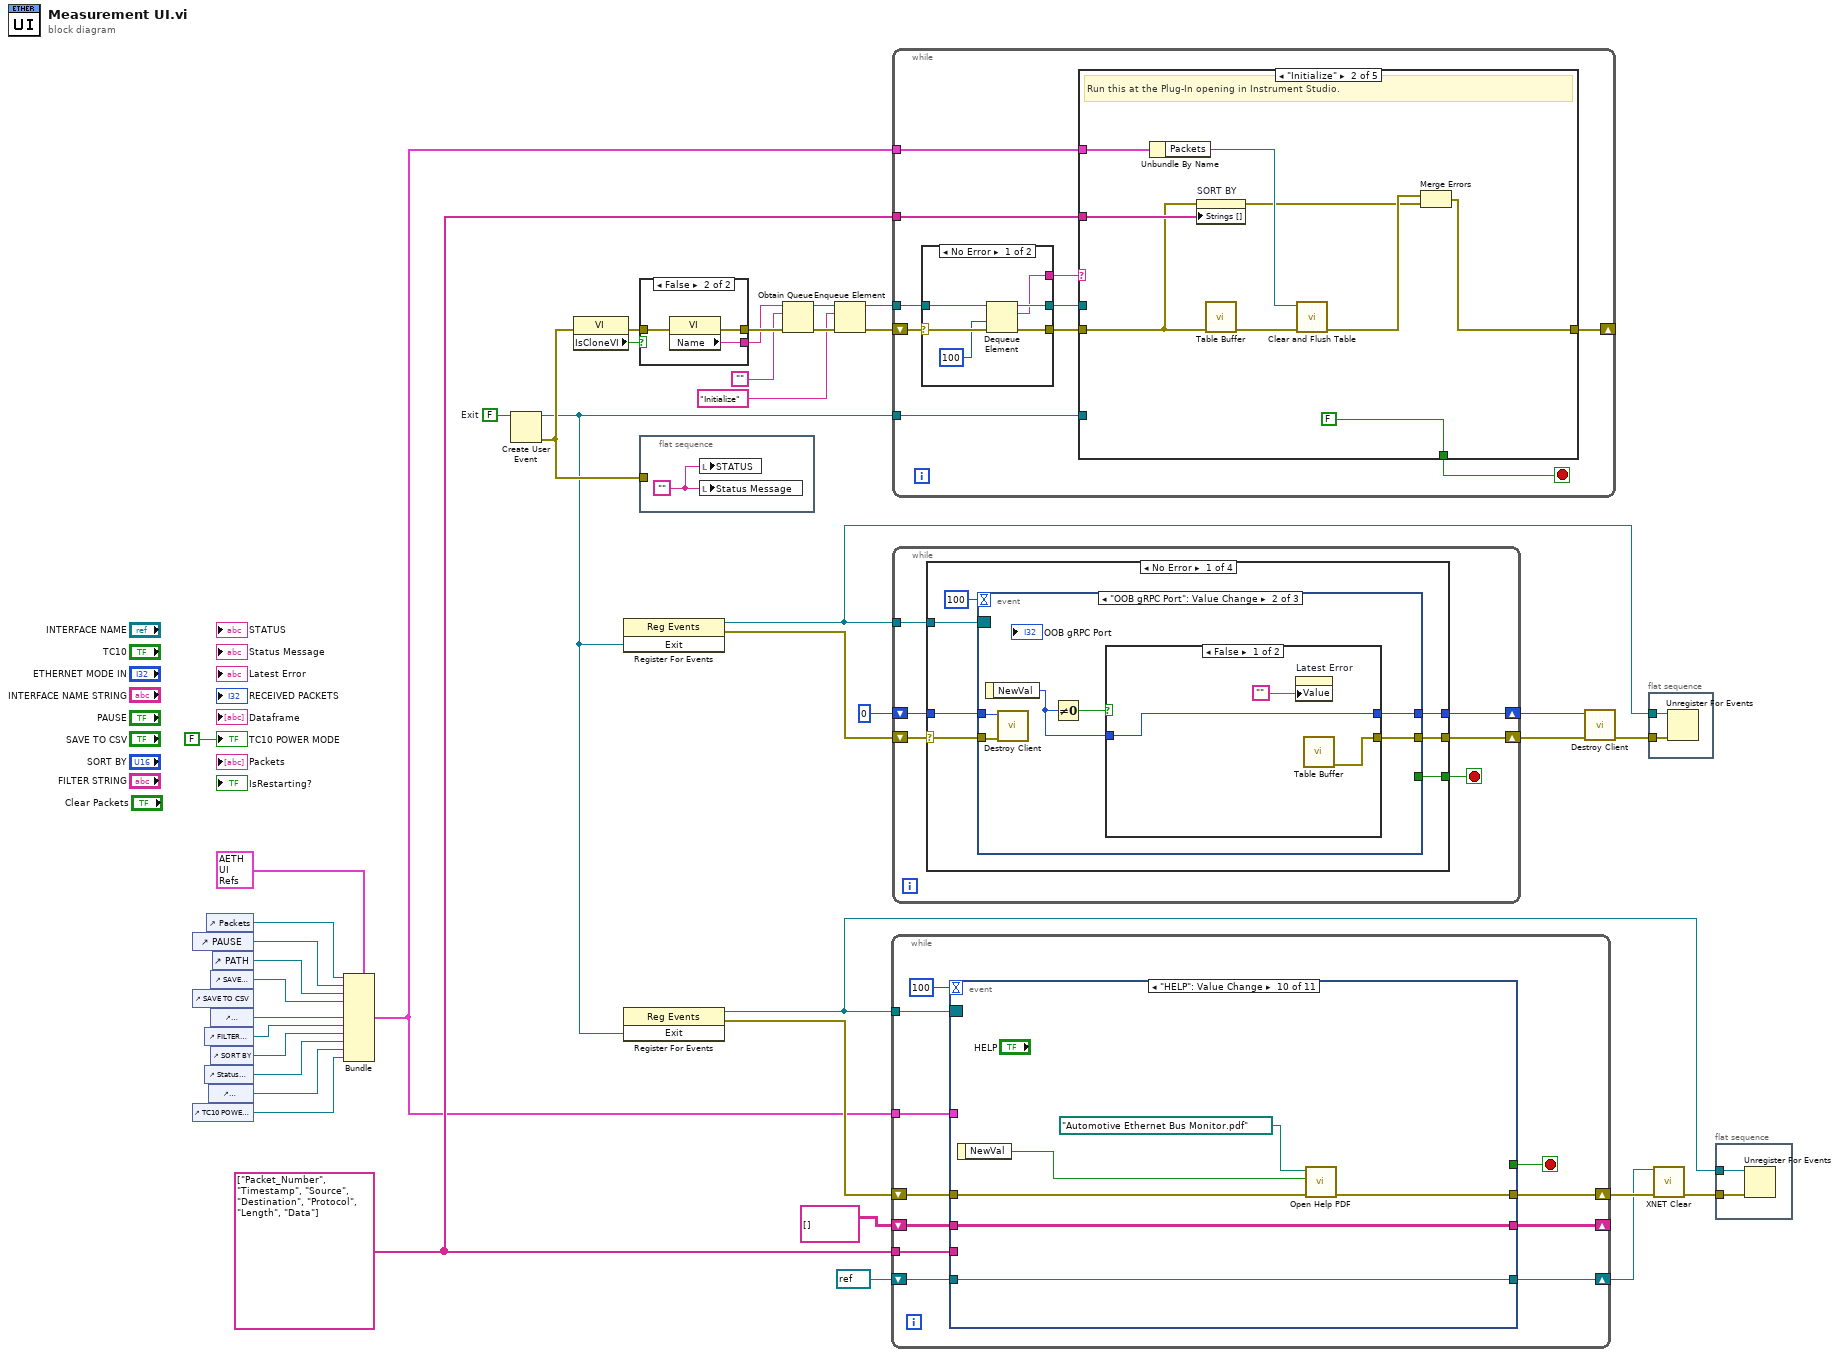
[diagram p0: block diagram]
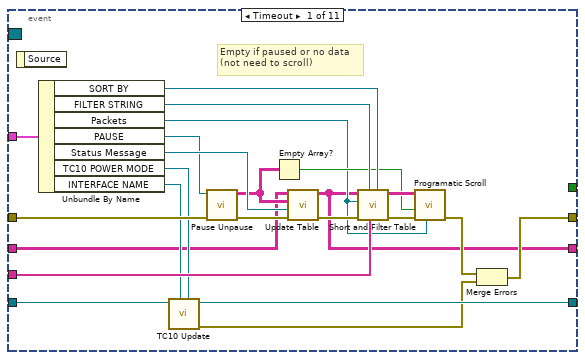
[diagram p2: hidden frame]
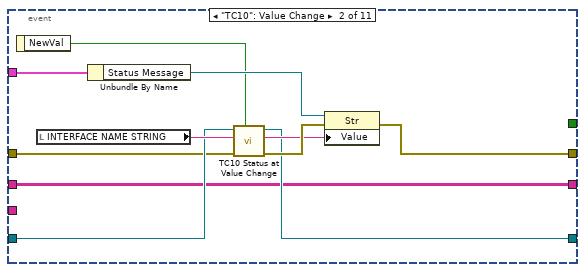
[diagram p3: hidden frame]
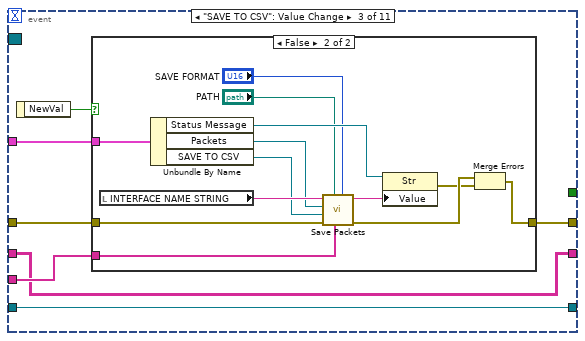
[diagram p4: hidden frame]
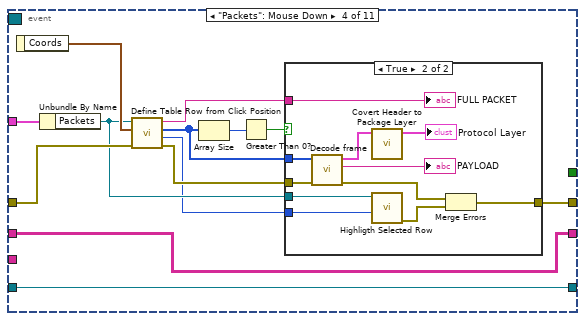
[diagram p6: hidden frame]
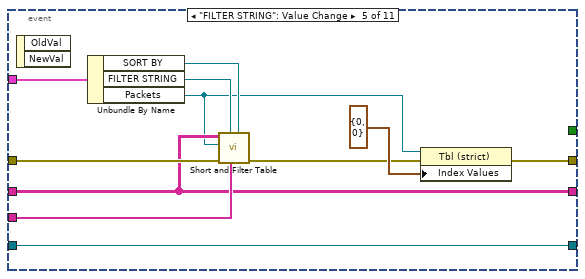
[diagram p8: hidden frame]
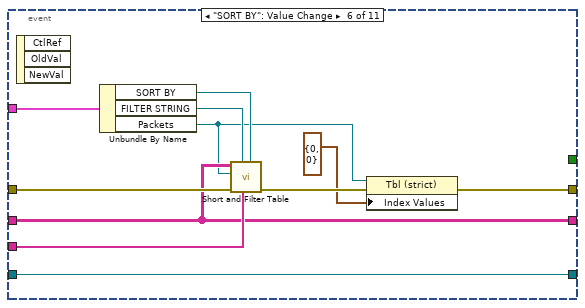
[diagram p9: hidden frame]
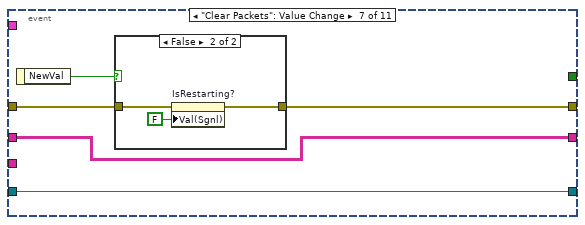
[diagram p10: hidden frame]
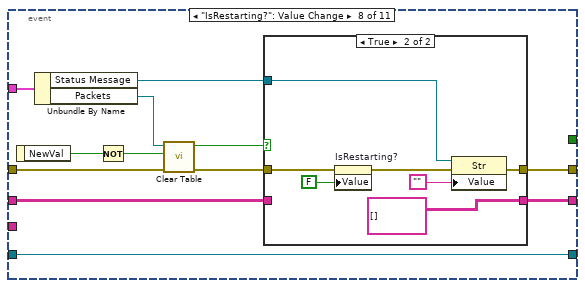
[diagram p12: hidden frame]
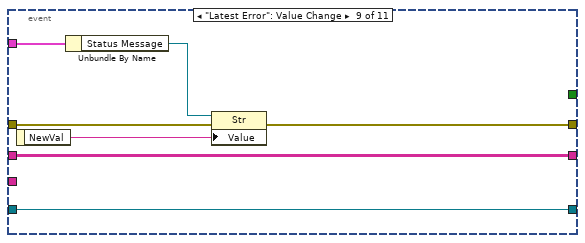
[diagram p14: hidden frame]
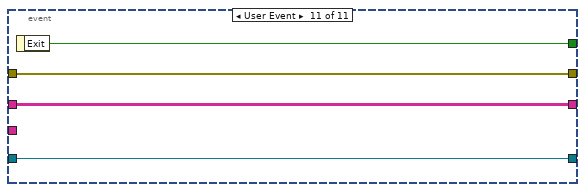
[diagram p15: hidden frame]
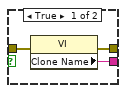
[diagram p16: hidden frame]
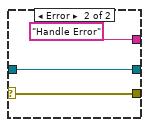
[diagram p17: hidden frame]
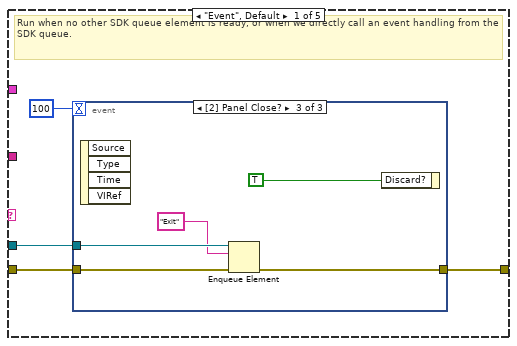
[diagram p18: hidden frame]
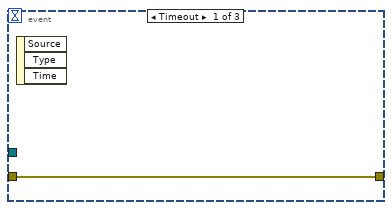
[diagram p19: hidden frame]
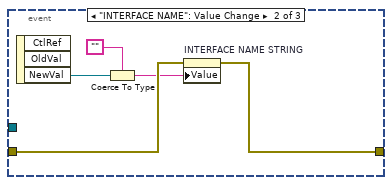
[diagram p20: hidden frame]
diagram:
  w30 = FALSE  # Exit
  w3 = string[] ["Packet_Number", "Timestamp", "Source", "Destination", "Protocol", "Length", "Data"] ("Headers")
  n1 = control-ref of="PAUSE"() -> (w17:refnum<vi>)
  n2 = control-ref of="SAVE TO CSV"() -> ()  [unwired: 1 out]
  n3 = control-ref of="TC10 POWER MODE"() -> (w10:refnum<vi>)
  n4 = control-ref of="FILTER STRING"() -> (w13:refnum<vi>)
  n5 = control-ref of="Status Message"() -> (w18:refnum<vi>)
  n6 = control-ref of="Packets"() -> (w19:refnum<vi>)
  n7 = control-ref of="INTERFACE NAME"() -> (w11:refnum<vi>)
  n8 = control-ref of="SAVE FORMAT"() -> (w15:refnum<vi>)
  n9 = control-ref of="ETHERNET MODE IN"() -> (w12:refnum<vi>)
  n10 = control-ref of="SORT BY"() -> (w14:refnum<vi>)
  n11 = control-ref of="PATH"() -> (w16:refnum<vi>)
  n12 = Bundle(cluster=T2 {"Packets"=refnum, "PAUSE"=refnum, "PATH "=refnum, "SAVE FORMAT"=refnum, "SAVE TO CSV"=refnum, "ETHERNET MODE IN"=refnum, "FILTER STRING"=refnum, "SORT BY"=refnum, "Status Message"=refnum, "INTERFACE NAME"=refnum, "TC10 POWER MODE"=refnum}, "Packets"=w19, "PAUSE"=w17, "PATH"=w16, "SAVE FORMAT"=w15, "ETHERNET MODE IN"=w12, "FILTER STRING"=w13, "SORT BY"=w14, "Status Message"=w18, "INTERFACE NAME"=w11, "TC10 POWER MODE"=w10) -> (w2:T2)  [unwired: 1 in]
  n13 = Create User Event(user event datatype=w30) -> (user event=w20:refnum<user-event>, error out=w25:errorcluster)  [unwired: 1 in]
  n14 = property class="VI"(error in=w25) -> (error out=w31:errorcluster, "IsCloneVI"=w32:bool)  [unwired: 1 in, 1 out]
  n15 = register-events(w20) -> (reference out=w28:refnum<event-registration>, error out=w27:errorcluster)  [unwired: 2 in]
  n16 = register-events(w20) -> (reference out=w21:refnum<event-registration>, error out=w4:errorcluster)  [unwired: 2 in]
  n17 = case shown="False" w32 {
    tunnel: [w43 w46] -> w40
    tunnel: [w42 w45] -> w39
    tunnel: w31 -> [w41 w44]
    frame True {
      n18 = property class="VI"(error in=w41) -> (error out=w43:errorcluster, "Clone Name"=w42:string)  [unwired: 1 in, 1 out]
    }
    frame False {
      n19 = property class="VI"(error in=w44) -> (error out=w46:errorcluster, "Name"=w45:string)  [unwired: 1 in, 1 out]
    }
  }
  n20 = flat-sequence {
    tunnel: w25 -> [_]
    frame #0 {
      w47 = ""
      n21 = local write "STATUS"(w47) -> ()
      n22 = local write "Status Message"(w47) -> ()
    }
  }
  n23 = Obtain Queue(name (unnamed)=w39, element data type="", error in (no error)=w40) -> (queue out=w36:refnum<queue>, error out=w38:errorcluster)  [unwired: 2 in, 1 out]
  n24 = Enqueue Element(queue=w36, element="Initialize", error in (no error)=w38) -> (queue out=w35:refnum<queue>, error out=w37:errorcluster)  [unwired: 1 in, 1 out]
  n25 = while {
    tunnel: w21 -> [w55]
    shift-right: [w56] -> w8
    shift-left: w4 -> [w58]
    tunnel: w2 -> [w53]
    shift-right: [w51] -> w7
    shift-left: refnum<k21> refnum ("XNET Refnum out") -> [w52]
    tunnel: w3 -> [w50]
    shift-right: [w48] -> _
    shift-left: string[][] [] ("Table Data in") -> [w49]
    stop <- w57 stop-if-true
    n26 = event shown="[9] \"HELP\": Value Change" {
      selector: w55 -> [_ _ _ _ _ _ _ _ _ _ _]
      dyn-events: _ -> [_ _ _ _ _ _ _ _ _ _ _]
      timeout: 100 -> [_ _ _ _ _ _ _ _ _ _ _]
      tunnel: [w76 w86 w96 w116 w147 w153 w164 w173 w194 w200 w206] -> w56
      tunnel: w58 -> [w78 w87 w99 w119 w145 w158 w165 w177 w193 w203 w206]
      tunnel: [_ _ _ _ _ _ _ _ _ _ w207] -> w57
      tunnel: w53 -> [w80 w89 w98 w126 w148 w157 _ w179 w197 _ _]
      tunnel: w52 -> [w79 w88 w97 w118 w146 w155 w162 w175 w192 w198 w205]
      tunnel: [w81 w84 w97 w118 w146 w155 w162 w175 w192 w198 w205] -> w51
      tunnel: w50 -> [w77 _ w95 _ w144 w156 _ _ _ _ _]
      tunnel: w49 -> [w61 w82 w93 w114 w140 w151 w161 w170 w191 w199 w204]
      tunnel: [w59 w82 w93 w114 w140 w151 w161 w174 w191 w199 w204] -> w48
      event Timeout {
        # "Empty if paused or no data\n(not need to scroll)"
        n27 = event-data() -> ()  [unwired: 1 in, 1 out]
        n28 = Unbundle By Name(w80) -> ("SORT BY"=w70:refnum<vi>, "FILTER STRING"=w71:refnum<vi>, "Packets"=w60:refnum<vi>, "PAUSE"=w72:refnum<vi>, "Status Message"=w73:refnum<vi>, "TC10 POWER MODE"=w75:refnum<vi>, "INTERFACE NAME"=w74:refnum<vi>)
        n29 = call "TC10 Update.vi"("TC10 State LED ref"=w75, "INTERFACE NAME ref"=w74, "XNET Session in"=w79) -> ("error out"=w63:errorcluster, "XNET Session out"=w81:refnum<k21>)  [unwired: 7 in]
        n30 = call "Pause Unpause.vi"("error in"=w78, "PauseUnpause Ref"=w72) -> ("error out"=w69:errorcluster, "New Data"=w62:string[][])  [unwired: 8 in]
        n31 = Empty Array?(array=w62) -> (empty?=w64:bool)
        n32 = call "Update Table.vi"("error in"=w69, "Status Message Ref"=w73, "New Data in"=w62, "Table Data in"=w61) -> ("error out"=w68:errorcluster, "Table Data out"=w59:string[][])  [unwired: 6 in]
        n33 = call "Short and Filter Table.vi"("Sort By Ref"=w70, "Headers"=w77, "Filter String Ref"=w71, "error in"=w68, "Table Ref"=w60, "Table Data"=w59) -> ("error out"=w67:errorcluster, "Sorted Table Data out"=w66:string[][])  [unwired: 4 in]
        n34 = call "Programatic Scroll.vi"("Table Ref"=w60, "error in"=w67, "Paused? (F)"=w64, "Packets"=w66) -> ("error out"=w65:errorcluster)  [unwired: 7 in]
        n35 = Merge Errors(w65, w63) -> (w76:errorcluster)
      }
      event "TC10": Value Change {
        n36 = event-data() -> ("NewVal"=w83:bool)  [unwired: 1 in]
        n37 = local read "INTERFACE NAME STRING"() -> (w92:string)
        n38 = Unbundle By Name(w89) -> ("Status Message"=w90:refnum<vi>)
        n39 = call "TC10 Status at Value Change.vi"("NewVal"=w83, "error in"=w87, "Interface Name String"=w92, "XNET Refnum in"=w88) -> ("error out"=w91:errorcluster, "Status Message String"=w85:string, "XNET Refnum out"=w84:refnum<k21>)  [unwired: 5 in]
        n40 = property class="Str"(reference=w90, error in=w91, "Value"=w85) -> (error out=w86:errorcluster)  [unwired: 1 out]
      }
      event "SAVE TO CSV": Value Change {
        n41 = event-data() -> ("NewVal"=w94:bool)  [unwired: 1 in]
        n42 = case shown="False" w94 {
          tunnel: w99 -> [w100 w113]
          tunnel: w98 -> [_ w111]
          tunnel: [w100 w107] -> w96
          tunnel: w95 -> [_ w102]
          frame True {
          }
          frame False {
            n43 = local read "INTERFACE NAME STRING"() -> (w112:string)
            n44 = Unbundle By Name(w111) -> ("Status Message"=w108:refnum<vi>, "Packets"=w109:refnum<vi>, "SAVE TO CSV"=w110:refnum<vi>)
            n45 = call "Save Packets.vi"("Save Format"="SAVE FORMAT", "Headers"=w102, "Path"="PATH", "error in"=w113, "SAVE TO CSV"=w110, "Packets"=w109, "Interface Name String"=w112) -> ("error out"=w106:errorcluster, "Status Message"=w104:string)  [unwired: 3 in]
            n46 = property class="Str"(reference=w108, "Value"=w104) -> (error out=w105:errorcluster)  [unwired: 1 in, 1 out]
            n47 = Merge Errors(w106, w105) -> (w107:errorcluster)
          }
        }
      }
      event "Packets": Mouse Down {
        n48 = event-data() -> ("Coords"=w120:T5)  [unwired: 1 in]
        n49 = Unbundle By Name(w126) -> ("Packets"=w117:refnum<vi>)
        n50 = call "Define Table Row from Click Position.vi"("error in"=w119, "Coords"=w120, "Table Ref"=w117) -> ("error out"=w125:errorcluster, "Current Row"=w115:i32, "Packet in Bytes"=w122:u8[], "Packet in String"=w124:string)  [unwired: 5 in]
        n51 = Array Size(array=w122) -> (size(s)=w121:i32)
        n52 = Greater Than 0?(x=w121) -> (x > 0?=w123:bool)
        n53 = case shown="True" w123 {
          tunnel: w122 -> [_ w137]
          tunnel: w124 -> [_ w133]
          tunnel: w125 -> [w127 w136]
          tunnel: [w127 w128] -> w116
          tunnel: w117 -> [_ w132]
          tunnel: w115 -> [_ w131]
          frame False {
          }
          frame True {
            n54 = call "Decode frame.vi"("error in (no error)"=w136, "frame data"=w137) -> ("error out"=w129:errorcluster, "Payload_String"=→"PAYLOAD":string, "Ethernet Header Cluster"=w138:T6)  [unwired: 7 in]
            n55 = call "Covert Header to Package Layer.vi"("Ethernet Header Cluster"=w138) -> ("Protocol Layer"=→"Protocol Layer":T1)  [unwired: 10 in]
            n56 = call "Highligth Selected Row.vi"("Current Row"=w131, "Table in"=w132) -> ("error out"=w130:errorcluster)  [unwired: 9 in]
            n57 = Merge Errors(w129, w130) -> (w128:errorcluster)
            "FULL PACKET" <- w133
          }
        }
      }
      event "FILTER STRING": Value Change {
        n58 = event-data() -> ()  [unwired: 1 in, 2 out]
        n59 = Unbundle By Name(w148) -> ("SORT BY"=w142:refnum<vi>, "FILTER STRING"=w143:refnum<vi>, "Packets"=w139:refnum<vi>)
        n60 = call "Short and Filter Table.vi"("Sort By Ref"=w142, "Headers"=w144, "Filter String Ref"=w143, "error in"=w145, "Table Ref"=w139, "Table Data"=w140) -> ("error out"=w141:errorcluster)  [unwired: 4 in, 1 out]
        n61 = property class="Tbl (strict)"(reference=w139, error in=w141, "Index Values"=T4 {"Row"=0, "Column"=0}) -> (error out=w147:errorcluster)  [unwired: 1 out]
      }
      event "SORT BY": Value Change {
        n62 = event-data() -> ()  [unwired: 1 in, 3 out]
        n63 = Unbundle By Name(w157) -> ("SORT BY"=w159:refnum<vi>, "FILTER STRING"=w160:refnum<vi>, "Packets"=w150:refnum<vi>)
        n64 = call "Short and Filter Table.vi"("Sort By Ref"=w159, "Headers"=w156, "Filter String Ref"=w160, "error in"=w158, "Table Ref"=w150, "Table Data"=w151) -> ("error out"=w154:errorcluster)  [unwired: 4 in, 1 out]
        n65 = property class="Tbl (strict)"(reference=w150, error in=w154, "Index Values"=T4 {"Row"=0, "Column"=0}) -> (error out=w153:errorcluster)  [unwired: 1 out]
      }
      event "Clear Packets": Value Change {
        n66 = event-data() -> ("NewVal"=w163:bool)  [unwired: 1 in]
        n67 = case shown="False" w163 {
          tunnel: w165 -> [w166 w169]
          tunnel: [w166 w168] -> w164
          frame True {
          }
          frame False {
            n68 = property on="IsRestarting?" class="Bool (strict)"(error in=w169, "Val(Sgnl)"=FALSE ("Value (Signaling)")) -> (error out=w168:errorcluster)  [unwired: 1 in, 1 out]
          }
        }
      }
      event "IsRestarting?": Value Change {
        n69 = event-data() -> ("NewVal"=w178:bool)  [unwired: 1 in]
        n70 = Unbundle By Name(w179) -> ("Status Message"=w172:refnum<vi>, "Packets"=w180:refnum<vi>)
        n71 = Not(x=w178) -> (.not. x?=w176:bool)
        n72 = call "Clear Table.vi"("error in"=w177, "Confirm? (F)"=w176, "Table in"=w180) -> ("error out"=w181:errorcluster, "T button?"=w171:bool)  [unwired: 7 in]
        n73 = case shown="True" w171 {
          tunnel: w181 -> [w182 w190]
          tunnel: [w183 string[][] [] ("Table Data in")] -> w174
          tunnel: [w182 w186] -> w173
          tunnel: w172 -> [_ w185]
          tunnel: w170 -> [w183 _]
          frame False {
          }
          frame True {
            n74 = property on="IsRestarting?" class="Bool (strict)"(error in=w190, "Value"=FALSE ("IsRestarting?")) -> (error out=w187:errorcluster)  [unwired: 1 in, 1 out]
            n75 = property class="Str"(reference=w185, error in=w187, "Value"="") -> (error out=w186:errorcluster)  [unwired: 1 out]
          }
        }
      }
      event "Latest Error": Value Change {
        n76 = event-data() -> ("NewVal"=w195:string)  [unwired: 1 in]
        n77 = Unbundle By Name(w197) -> ("Status Message"=w196:refnum<vi>)
        n78 = property class="Str"(reference=w196, error in=w193, "Value"=w195) -> (error out=w194:errorcluster)  [unwired: 1 out]
      }
      event "HELP": Value Change {
        n79 = event-data() -> ("NewVal"=w202:bool)  [unwired: 1 in]
        n80 = call "Open Help PDF.vi"("error in"=w203, "NewVal"=w202, "Path after documentation"=path "Automotive Ethernet Bus Monitor.pdf") -> ("error out"=w200:errorcluster)  [unwired: 8 in]
      }
      event User Event {
        n81 = event-data() -> ("Exit"=w207:bool)  [unwired: 1 in]
      }
    }
  }
  n82 = while {
    shift-right: [w212] -> _
    shift-left: w37 -> [w217]
    tunnel: w35 -> [w215]
    tunnel: w20 -> [w210]
    tunnel: w2 -> [w209]
    tunnel: w3 -> [w208]
    stop <- w211 stop-if-true
    n83 = case shown="No Error" w217 {
      selector: w217 -> [w223 w226]
      tunnel: [w222 w226] -> w216
      tunnel: w215 -> [w221 w225]
      tunnel: [w220 w225] -> w214
      tunnel: [w219 "Handle Error"] -> w213
      frame No Error {
        n84 = Dequeue Element(queue=w221, timeout in ms (-1)=100, error in (no error)=w223) -> (queue out=w220:refnum<queue>, element=w219:string, error out=w222:errorcluster)  [unwired: 1 out]
      }
      frame Error {
      }
    }
    n85 = case shown="\"Initialize\"" w213 {
      tunnel: w216 -> [w230 w244 w252 w276 w277]
      tunnel: w214 -> [w228 _ _ w274 _]
      tunnel: [w227 w245 w252 w266 w277] -> w212
      tunnel: [_ FALSE _ TRUE _] -> w211
      tunnel: w210 -> [_ _ _ w268 _]
      tunnel: w209 -> [_ w248 _ _ _]
      tunnel: w208 -> [_ w247 _ _ _]
      frame "Event", Default {
        # "Run when no other SDK queue element is ready, or when we directly call an event handling from the SDK queue."
        n86 = event shown="[2] Panel Close?" {
          selector: _ -> [_ _ _]
          dyn-events: _ -> [_ _ _]
          timeout: 100 -> [_ _ _]
          tunnel: w230 -> [w231 w236 w240]
          tunnel: w228 -> [_ _ w238]
          tunnel: [w231 w235 w239] -> w227
          event Timeout {
            n87 = event-data() -> ()  [unwired: 1 in, 3 out]
          }
          event "INTERFACE NAME": Value Change {
            n88 = event-data() -> ("NewVal"=w234:refnum<k21>)  [unwired: 1 in, 2 out]
            n89 = Coerce To Type(0:w234, 1:"") -> (2:w232:string)
            n90 = property on="INTERFACE NAME STRING" class="Str"(error in=w236, "Value"=w232) -> (error out=w235:errorcluster)  [unwired: 1 in, 1 out]
          }
          event Panel Close? {
            n91 = event-data() -> ()  [unwired: 1 in, 4 out]
            n92 = Enqueue Element(queue=w238, element="Exit", error in (no error)=w240) -> (error out=w239:errorcluster)  [unwired: 1 in, 2 out]
            n93 = event-data("Discard?"=TRUE) -> ()  [unwired: 1 in, 1 out]
          }
        }
      }
      frame "Initialize" {
        # "Run this at the Plug-In opening in Instrument Studio."
        n94 = Unbundle By Name(w248) -> ("Packets"=w243:refnum<vi>)
        n95 = property on="SORT BY" class="Ring (strict)"(error in=w244, "Strings []"=w247) -> (error out=w242:errorcluster)  [unwired: 1 in, 1 out]
        n96 = call-poly "Table Buffer.vi"("error in (no error)"=w244) -> ("error out"=w249:errorcluster)  [unwired: 10 in]
        n97 = call "Clear and Flush Table.vi"("error in"=w249, "Table in"=w243) -> ("error out"=w246:errorcluster)  [unwired: 9 in]
        n98 = Merge Errors(w246, w242) -> (w245:errorcluster)
      }
      frame "Post UI Update" {
        # "This case will be triggered, after framework updates the User interface with result values."
        n99 = local read "OOB gRPC Port"() -> (w256:i32)
        n100 = local read "Latest Error"() -> (w251:string)
        n101 = local read "STATUS"() -> (w254:string)
        n102 = feedback #1(0 ("OOB gRPC Port")) -> (w258:i32)
        n103 = feedback-in #1(w256) -> ()
        n104 = Not Equal?(x=w254, y=w251) -> (x != y?=w255:bool)
        n105 = Not Equal?(x=w256, y=w258) -> (x != y?=w259:bool)
        n106 = Not Equal To 0?(x=w256) -> (x != 0?=w260:bool)
        n107 = case shown="True" w255 {
          tunnel: w254 -> [_ w262]
          frame False {
          }
          frame True {
            n108 = property on="Latest Error" class="Str"("Val(Sgnl)"=w262) -> ()  [unwired: 2 in, 2 out]
          }
        }
        n109 = Compound Arithmetic op=AND(w260, w259) -> (w257:bool)
        n110 = case shown="True" w257 {
          tunnel: w256 -> [_ w263]
          frame False {
          }
          frame True {
            n111 = property on="OOB gRPC Port" class="DigNum (strict)"("Val(Sgnl)"=w263) -> ()  [unwired: 2 in, 2 out]
          }
        }
        n112 = Wait (ms)(milliseconds to wait=u32 100) -> ()  [unwired: 1 out]
      }
      frame "Exit" {
        # "This case is triggered to close the User Interface from framework."
        n113 = call-poly "Table Buffer.vi"() -> ("error out"=w264:errorcluster)  [unwired: 11 in]
        n114 = Flush Queue(queue=w274, error in (no error)=w276) -> (queue out=w273:refnum<queue>, error out=w272:errorcluster)  [unwired: 1 out]
        n115 = Generate User Event(user event=w268, event data cluster=TRUE ("event data")) -> (user event out=w269:refnum<user-event>)  [unwired: 2 in, 1 out]
        n116 = Release Queue(queue=w273, force destroy? (F)=TRUE, error in (no error)=w272) -> (error out=w267:errorcluster)  [unwired: 2 out]
        n117 = Destroy User Event(user event=w269) -> (error out=w265:errorcluster)  [unwired: 1 in]
        n118 = Merge Errors(w264, w267, w265) -> (w266:errorcluster)
      }
      frame "Handle Error" {
      }
    }
  }
  n119 = while {
    tunnel: w28 -> [w280]
    shift-right: [w281] -> w24
    shift-left: w27 -> [w283]
    shift-right: [w278] -> w29
    shift-left: T3 0 ("gRPC ID out") -> [w279]
    stop <- w282 stop-if-true
    n120 = case shown="No Error" w283 {
      selector: w283 -> [w288 w322 _ _]
      tunnel: [w285 TRUE w333 w343] -> w282
      tunnel: [w289 w322 errorcluster {"status"=FALSE, "code"=0, "source"=""} ("error IO") errorcluster {"status"=FALSE, "code"=0, "source"=""} ("error IO")] -> w281
      tunnel: w280 -> [w290 _ _ _]
      tunnel: w279 -> [w287 w328 w331 w341]
      tunnel: [w286 w328 w331 w341] -> w278
      frame No Error {
        n121 = event shown="[1] \"OOB gRPC Port\": Value Change" {
          selector: w290 -> [_ _ _]
          dyn-events: _ -> [_ _ _]
          timeout: 100 -> [_ _ _]
          tunnel: [w293 w305 w318] -> w289
          tunnel: w288 -> [w298 w302 w318]
          tunnel: w287 -> [w299 w303 w319]
          tunnel: [w295 w304 w319] -> w286
          tunnel: [_ _ w320] -> w285
          event Timeout {
            n122 = event-data() -> ()  [unwired: 1 in, 1 out]
            n123 = call "Get Data Client Wrapper.vi"("error in"=w298, "gRPC ID in"=w299) -> ("error out"=w297:errorcluster, "Payload"=w296:u8[], "gRPC ID out"=w295:T3)  [unwired: 7 in]
            n124 = call "Convert and Enqueue.vi"("error in"=w297, "Data"=w296) -> ("error out"=w294:errorcluster)  [unwired: 8 in, 1 out]
            n125 = call-poly "Table Buffer.vi"("error in"=w294) -> ("error out"=w293:errorcluster, "Messages"=w292:i32)  [unwired: 9 in]
            n126 = Greater Than 0?(x=w292) -> (x > 0?=→"New Data?":bool)
          }
          event "OOB gRPC Port": Value Change {
            n127 = event-data() -> ("NewVal"=w301:i32)  [unwired: 1 in]
            n128 = call "Destroy Client.vi"("error in"=w302, "gRPC ID"=w303) -> ()  [unwired: 9 in, 1 out]
            n129 = Not Equal To 0?(x=w301) -> (x != 0?=w300:bool)
            n130 = case shown="False" w300 {
              tunnel: [w307 w310] -> w305
              tunnel: w301 -> [w308 w315]
              tunnel: [w308 w314] -> w304
              frame False {
                n131 = property on="Latest Error" class="Str"("Value"="") -> ()  [unwired: 2 in, 2 out]
                n132 = call-poly "Table Buffer.vi"() -> ("error out"=w307:errorcluster)  [unwired: 11 in]
              }
              frame True {
                n133 = control-ref of="IsRestarting?"() -> (w309:refnum<vi>)
                n134 = Format Into String(w315) -> (resulting string=w317:string)  [unwired: 3 in, 1 out]
                n135 = Concatenate Strings("localhost:" ("string"), w317) -> (w313:string)
                n136 = call "Create Client.vi"("address"=w313) -> ("error out"=w312:errorcluster, "gRPC ID Out"=w314:T3)  [unwired: 9 in]
                n137 = call "Set and Wait to Completion.vi"("Bool Ref"=w309) -> ("error out"=w311:errorcluster)  [unwired: 10 in]
                n138 = Merge Errors(w312, w311) -> (w310:errorcluster)
              }
            }
          }
          event User Event {
            n139 = event-data() -> ("Exit"=w320:bool)  [unwired: 1 in]
          }
        }
      }
      frame Default {
        n140 = Wait (ms)(milliseconds to wait=u32 5000) -> ()  [unwired: 1 out]
        n141 = Unbundle By Name(w322) -> ("code"=w327:i32, "source"=w326:string)
        n142 = Format Into String(initial string="OOB gRPC client loop stopped, Error:" ("format string"), w327, "\r\n", w326) -> (resulting string=w323:string)  [unwired: 2 in, 1 out]
        n143 = local write "Status Message"(w323) -> ()
      }
      frame Error {
        n144 = local read "OOB gRPC Port"() -> (w335:i32)
        n145 = Wait (ms)(milliseconds to wait=u32 100) -> ()  [unwired: 1 out]
        n146 = Equal?(x=w335, y=-1 ("x")) -> (x = y?=w333:bool)
        n147 = case shown="False" w333 {
          selector: w333 -> [w336 _]
          tunnel: w335 -> [_ _]
          frame False {
            n148 = property on="OOB gRPC Port" class="DigNum (strict)"("Val(Sgnl)"=0 ("Value (Signaling)")) -> ()  [unwired: 2 in, 2 out]
            "CAPTURING STREAM" <- w336
          }
          frame True {
            n149 = local write "Status Message"("OOB gRPC server side Error.\nMeasurement Logic didn't get the gRPC port from OOB server.\nRestart the plugin." ("Status")) -> ()
          }
        }
      }
      frame Error {
        n150 = local read "OOB gRPC Port"() -> (w345:i32)
        n151 = Wait (ms)(milliseconds to wait=u32 2000) -> ()  [unwired: 1 out]
        n152 = Equal?(x=w345, y=-1 ("x")) -> (x = y?=w343:bool)
        n153 = case shown="False" w343 {
          tunnel: w345 -> [w346 _]
          tunnel: ["Reconnecting..." ("Status") "OOB gRPC server side Error.\nMeasurement Logic didn't get the gRPC port from OOB server.\nRestart the plugin." ("Status")] -> w339
          frame False {
            n154 = property on="OOB gRPC Port" class="DigNum (strict)"("Val(Sgnl)"=w346) -> ()  [unwired: 2 in, 2 out]
          }
          frame True {
          }
        }
        n155 = local write "Status Message"(w339) -> ()
      }
    }
  }
  n156 = call "Destroy Client.vi"("error in"=w24, "gRPC ID"=w29) -> ("error out"=w23:errorcluster)  [unwired: 9 in]
  n157 = flat-sequence {
    tunnel: w28 -> [w350]
    tunnel: w23 -> [w349]
    frame #0 {
      n158 = Unregister For Events(event registration refnum=w350, error in=w349) -> ()  [unwired: 1 out]
    }
  }
  n159 = call <vilib>:"XNET Clear.vi"("session in"=w7, "error in (no error)"=w8) -> ("error out"=w6:errorcluster)  [unwired: 13 in]
  n160 = flat-sequence {
    tunnel: w21 -> [w352]
    tunnel: w6 -> [w351]
    frame #0 {
      n161 = Unregister For Events(event registration refnum=w352, error in=w351) -> ()  [unwired: 1 out]
    }
  }
  "TC10 POWER MODE" <- FALSE ("TC10 POWER MODE")
